vi "FixJKIHelper.vi"() -> ()   [LabVIEW 2017]
uses:
  _Support/Common/Format Timestamp.vi
  _Shared/CSM Shared.lvlib
  _csmDoc/csmdoc.lvlib
  Communicable State Machine.lvlib
  user32.dll
panel:
  out "String Cache":string
  in  "Bottom Right":string
  in  "Bottom Left":string
  out "2D Picture":picture
  in  "Error in":errorcluster caption="error in (no error)"
  out "Listbox":i32(listbox)
  in  "Progress Bar":u8(slide) scale=-1.0..226.0
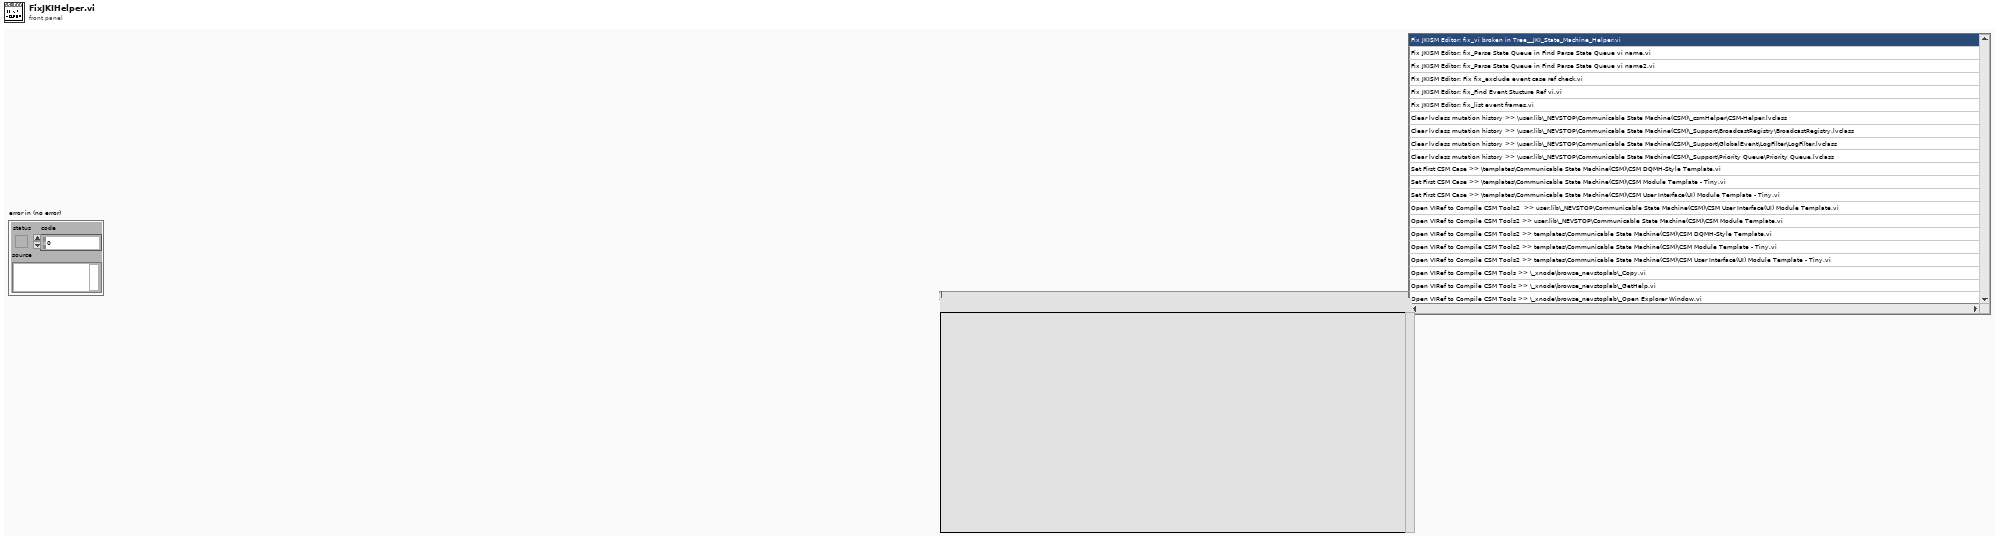
[diagram p1: front panel]
types:
  T1 = enum32{"Invalid", "Standard", "Closed", "Hidden", "Minimized", "Maximized"}
  T2 = enum32{"invalid app kind", "Development System", "Run Time System", "Student Edition", "Embedded LabVIEW", "Evaluation", "Custom"}
  T3 = cluster{"Core":cluster{"Current VI Reference":refnum<vi>, "Close Panel on Exit?":bool}, "Listbox Symbols":i32[], "Listbox Index":i32, "_JKI State Machine Helper VIs":path[], "CSM Templates":path[], "CSM lvclass":path[], "_JKI State Machine Helper Folders":path[], "Actions":string[], "LangID":string, "DescMap":variant, "NoteMap":variant, "Polish":cluster{"Version":refnum<vi>, "Action":refnum<vi>, "Progress Bar":refnum<vi>, "2D Picture":refnum<vi>, "Hold":bool, "Slides":picture[]}}
  T4 = cluster{"Version":refnum<vi>, "Action":refnum<vi>, "Progress Bar":refnum<vi>, "2D Picture":refnum<vi>, "Hold":bool, "Slides":picture[]}
  T5 = cluster{"Current VI Reference":refnum<vi>, "Close Panel on Exit?":bool}
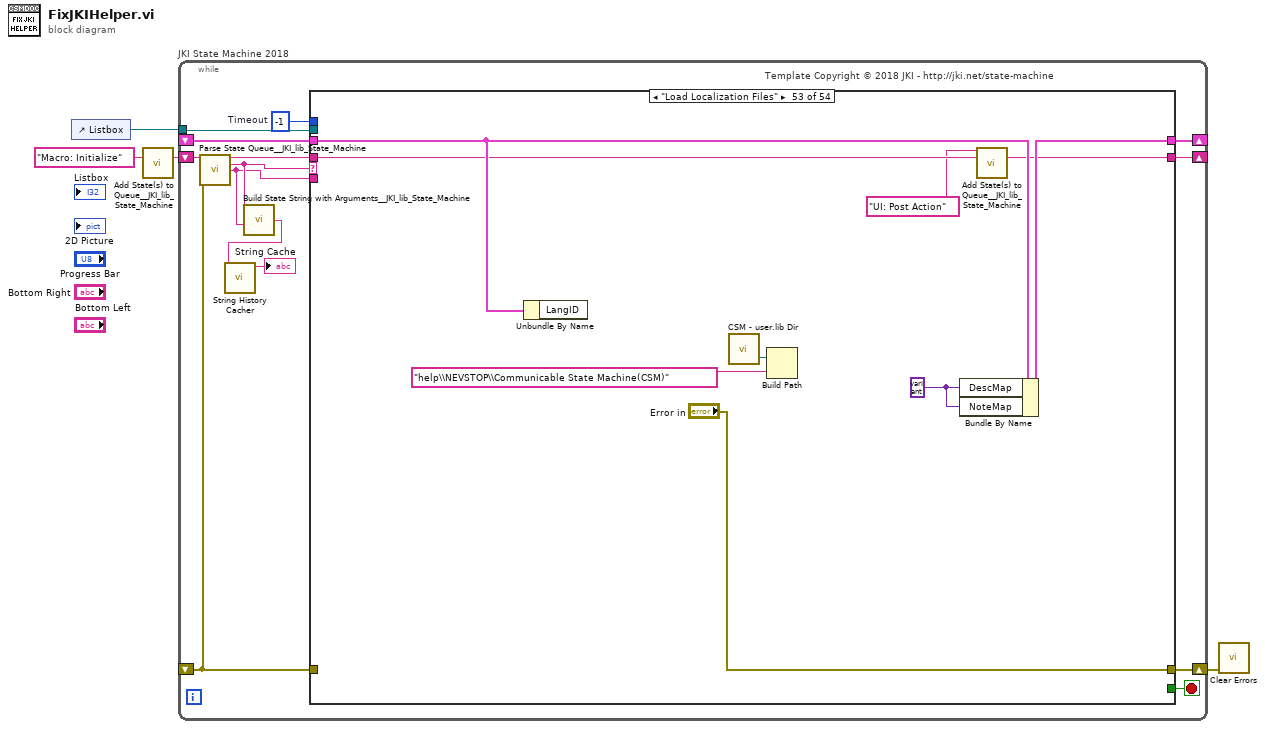
[diagram p0: block diagram]
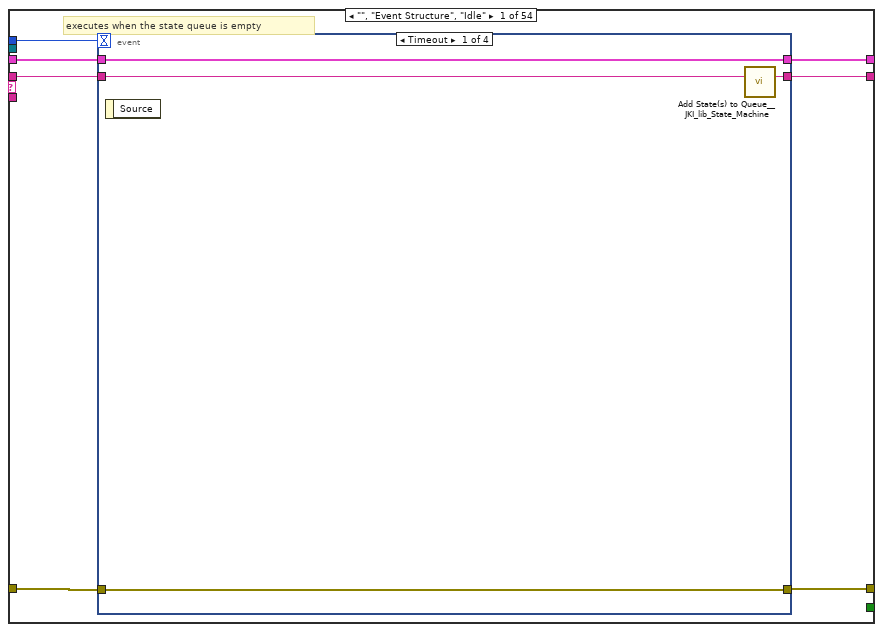
[diagram p2: hidden frame]
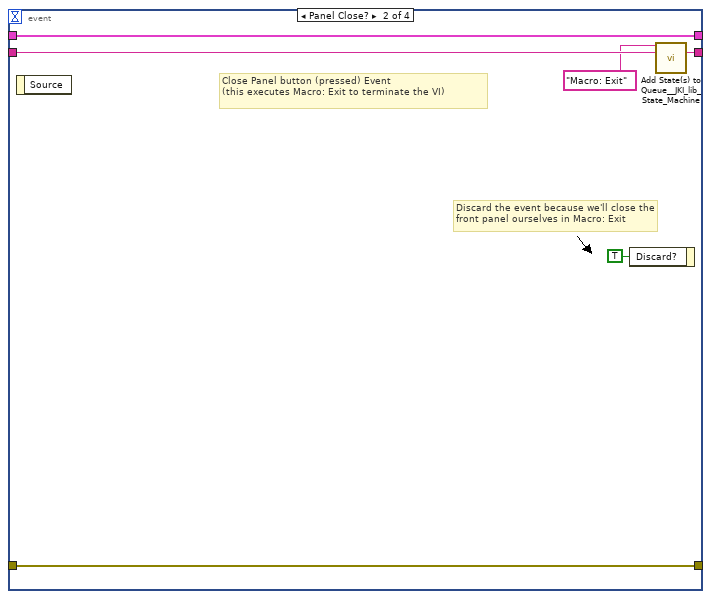
[diagram p3: hidden frame]
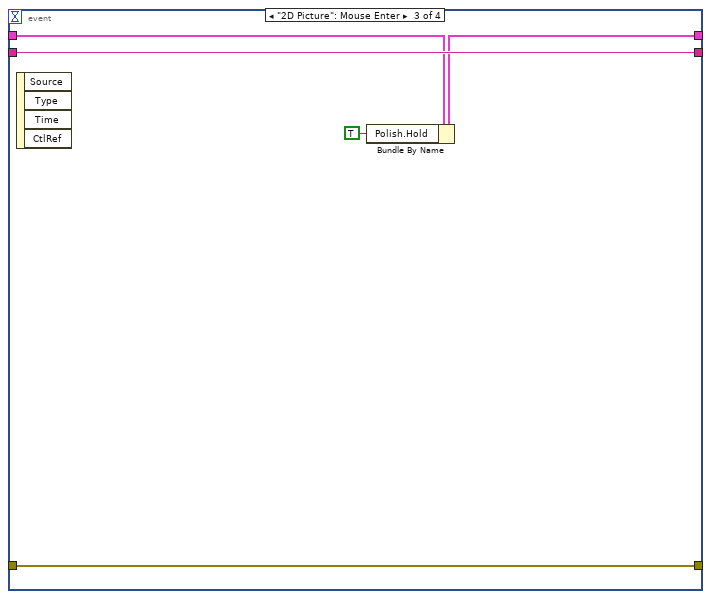
[diagram p4: hidden frame]
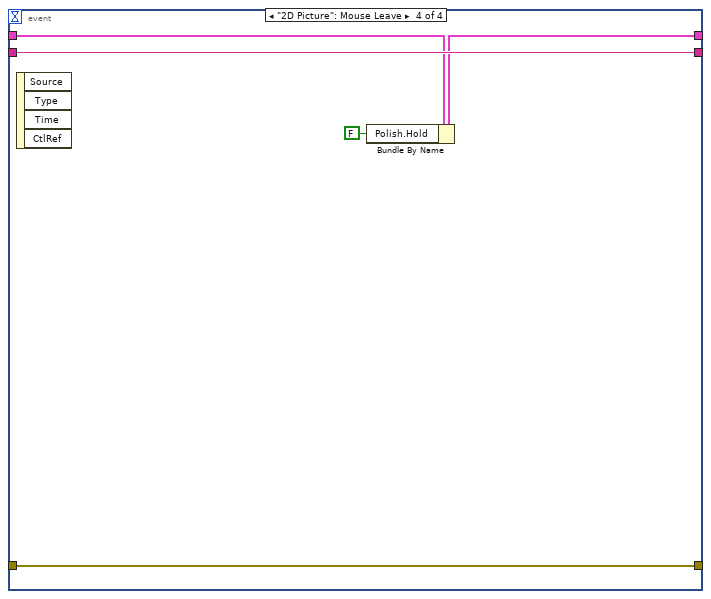
[diagram p5: hidden frame]
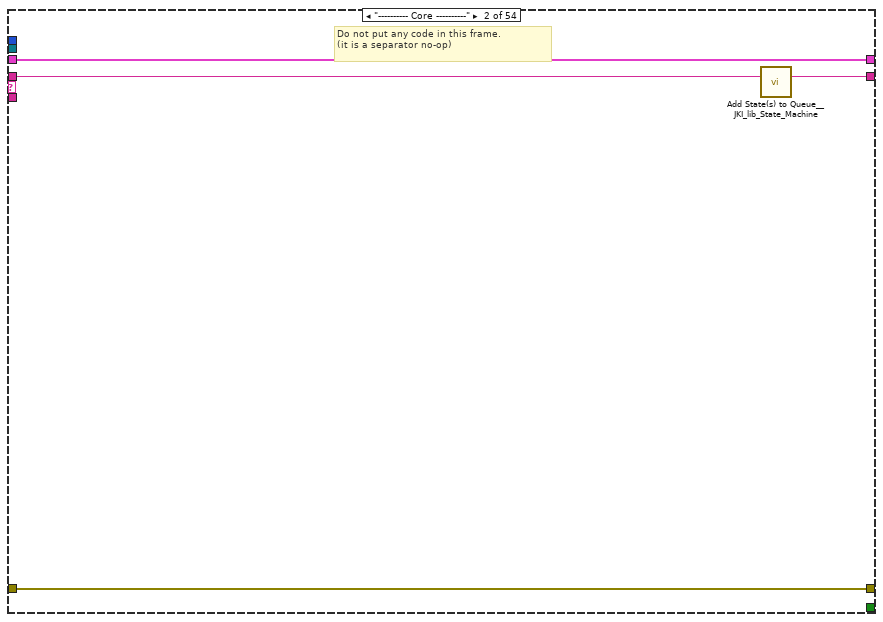
[diagram p6: hidden frame]
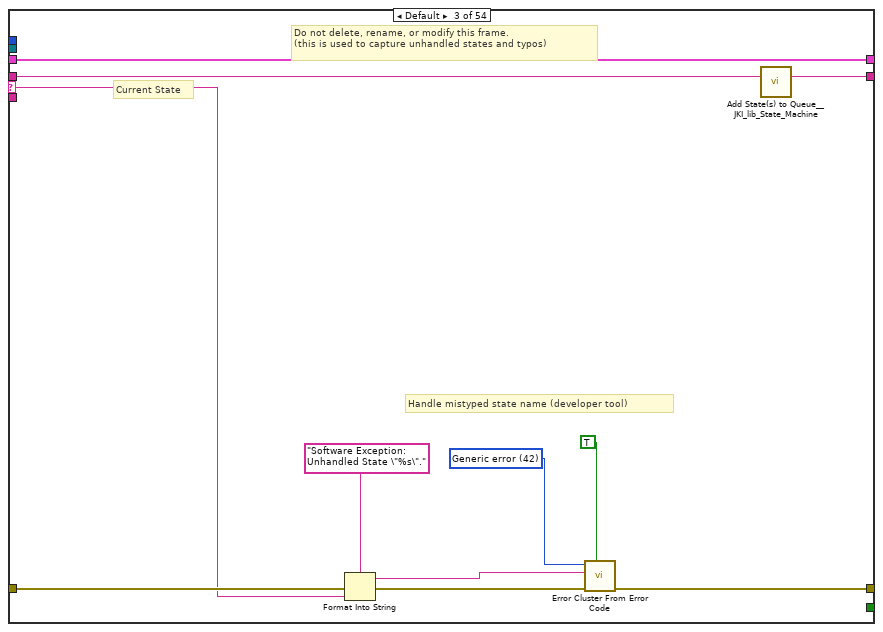
[diagram p7: hidden frame]
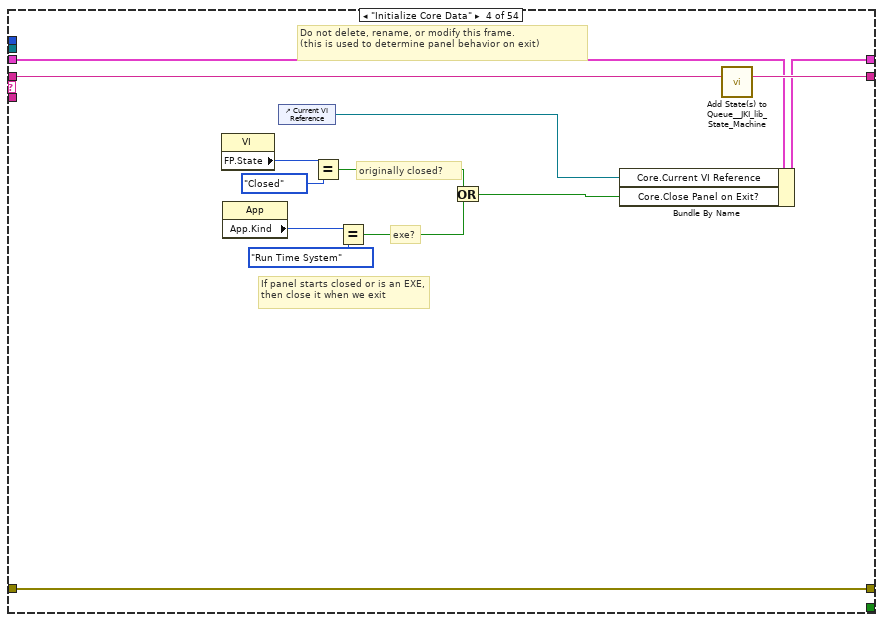
[diagram p8: hidden frame]
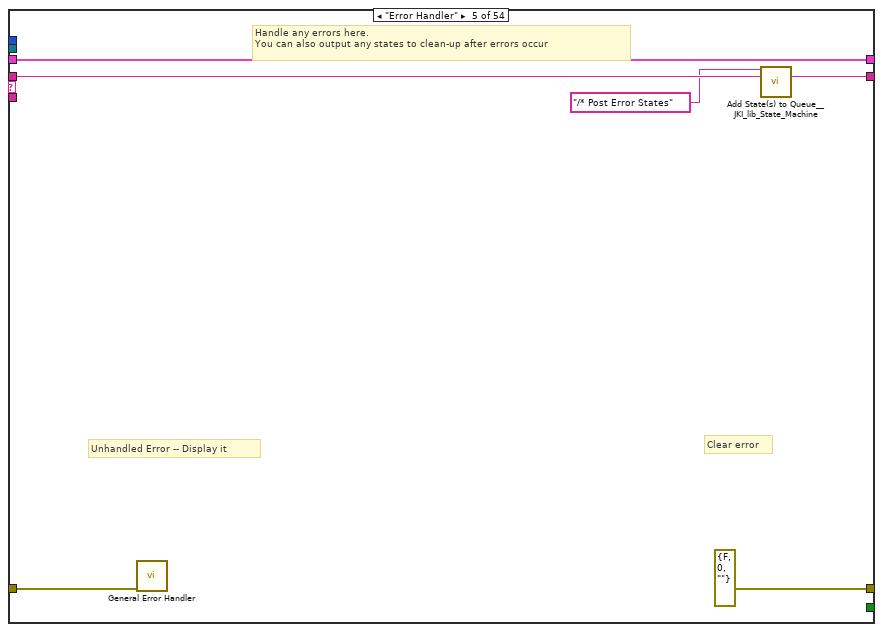
[diagram p9: hidden frame]
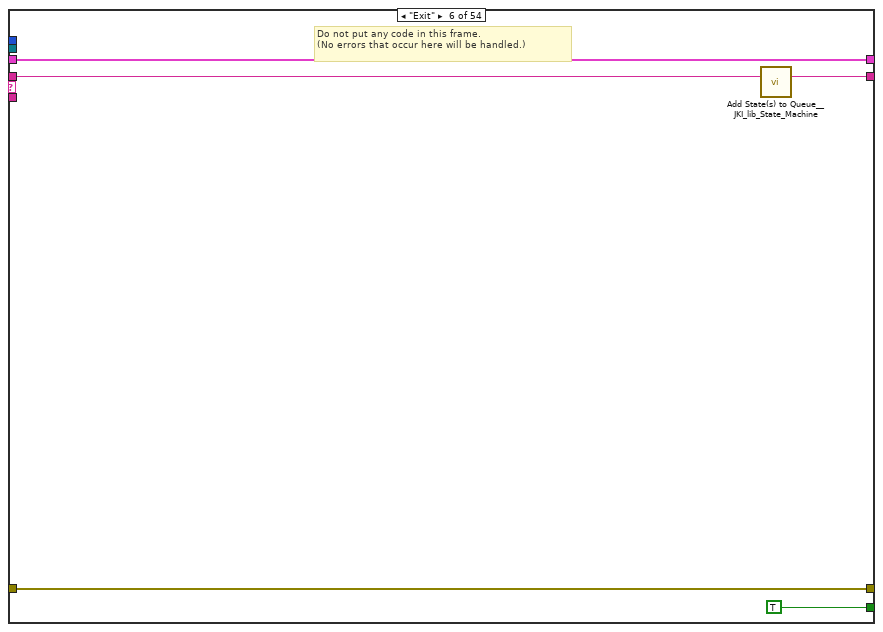
[diagram p10: hidden frame]
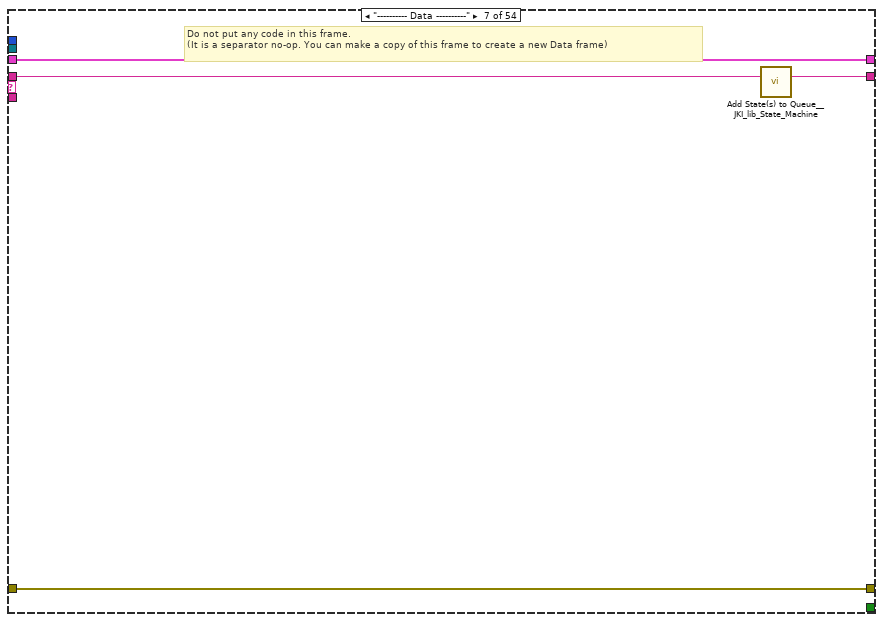
[diagram p11: hidden frame]
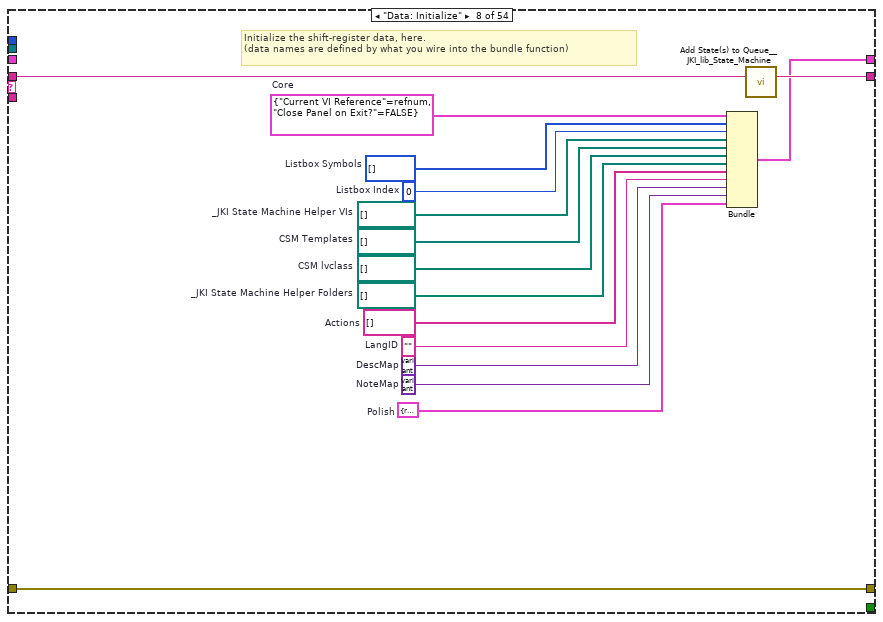
[diagram p12: hidden frame]
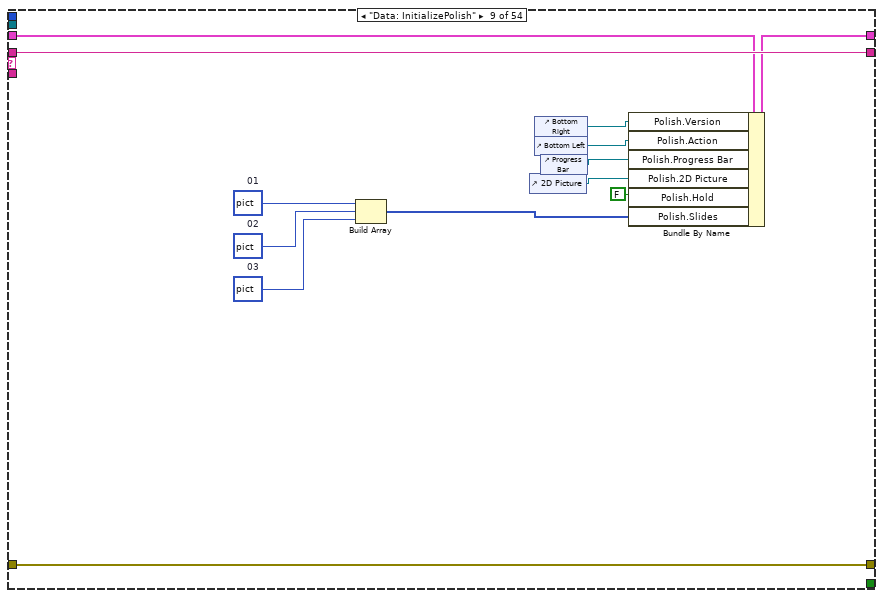
[diagram p13: hidden frame]
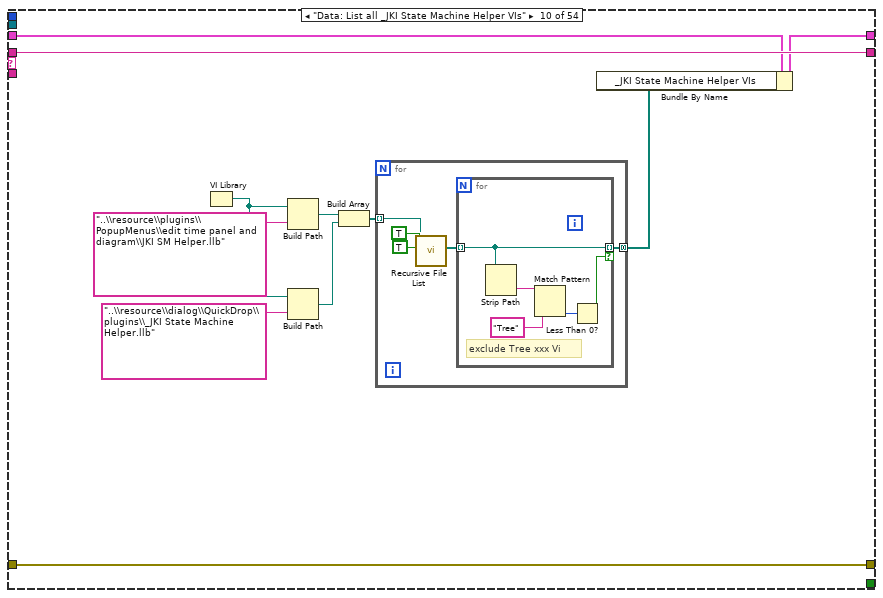
[diagram p14: hidden frame]
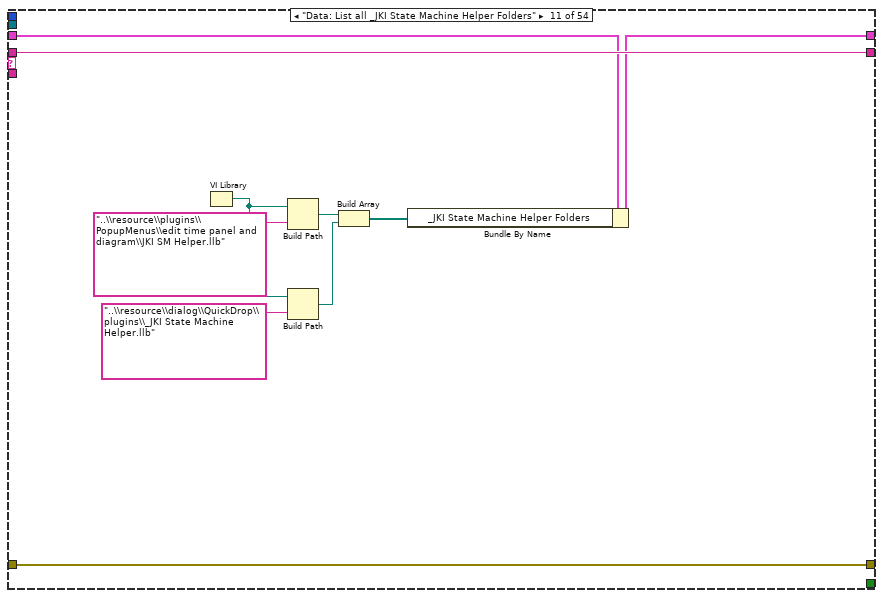
[diagram p15: hidden frame]
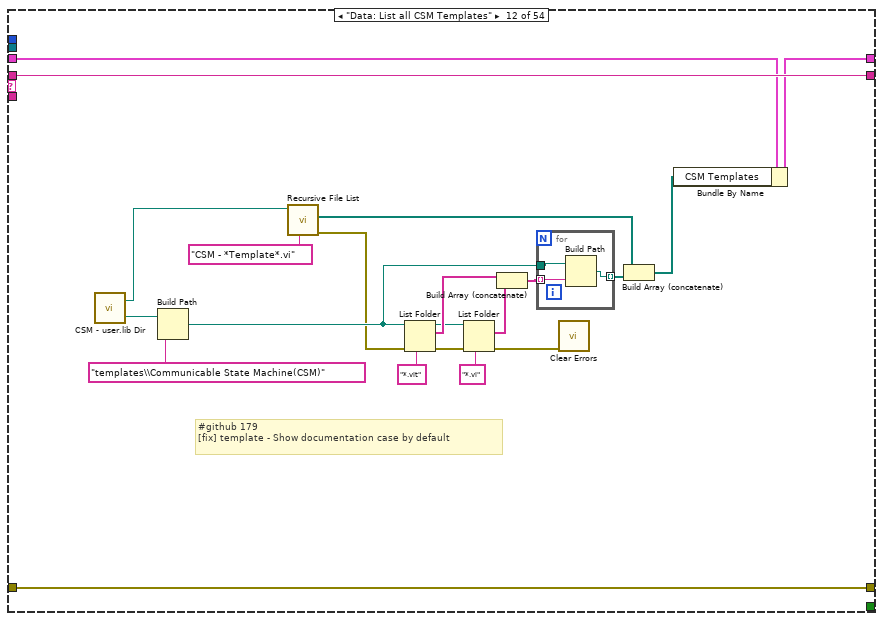
[diagram p16: hidden frame]
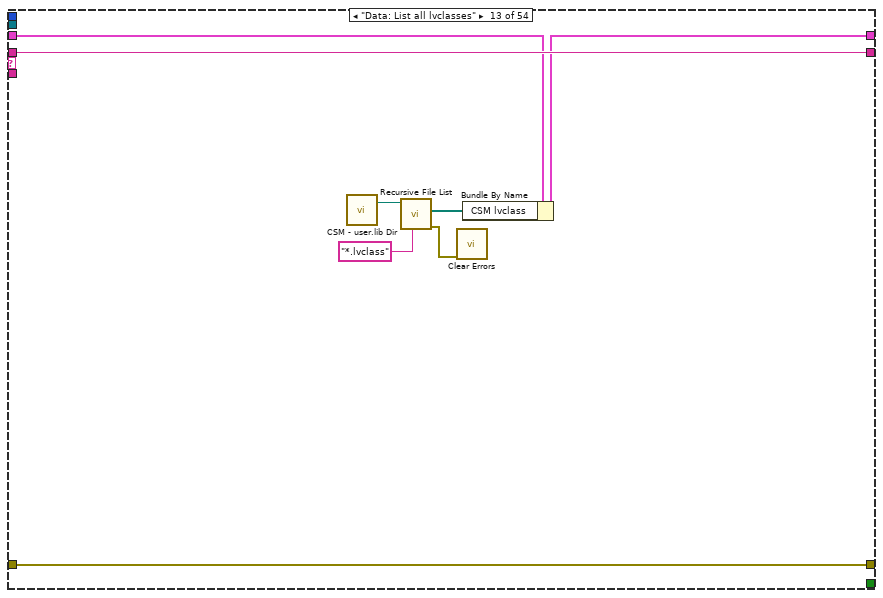
[diagram p17: hidden frame]
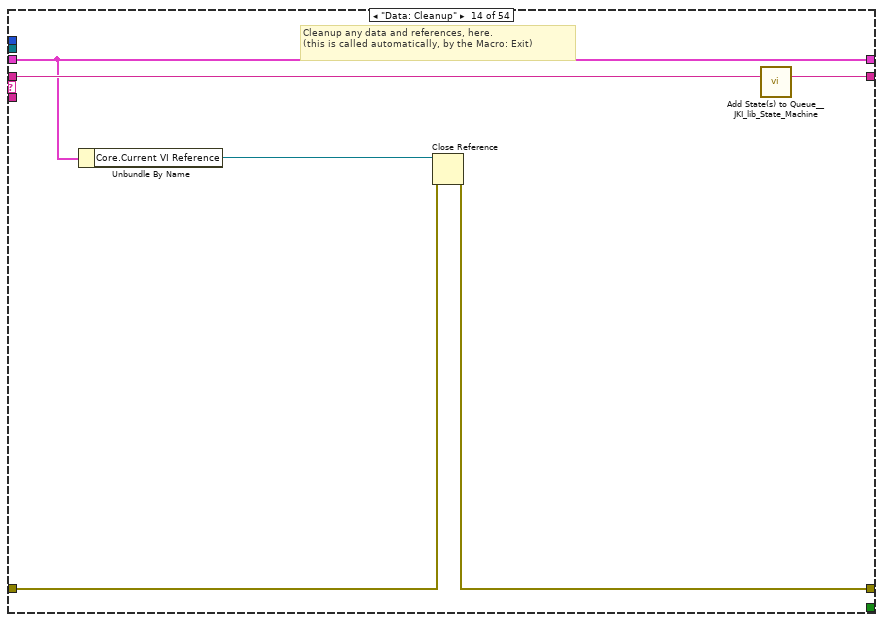
[diagram p18: hidden frame]
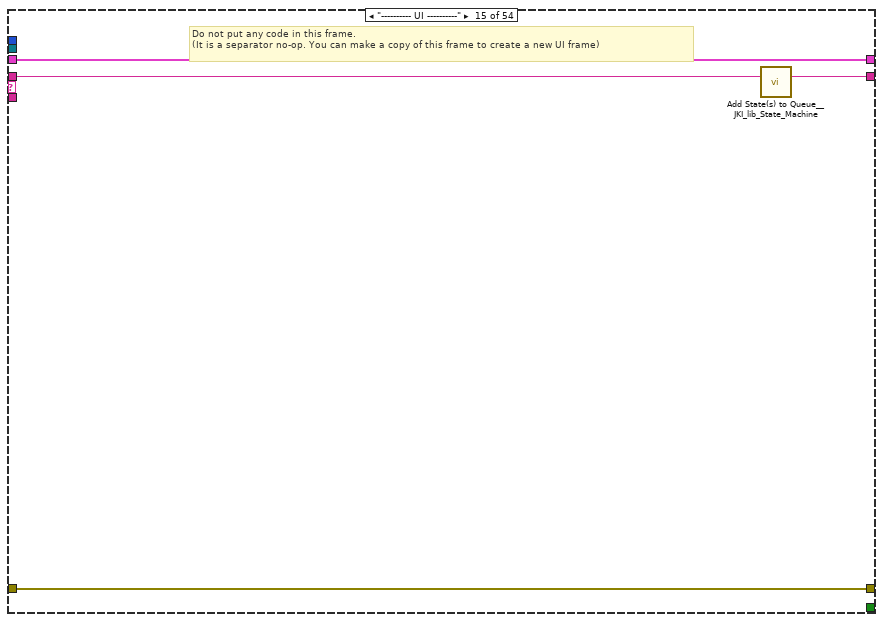
[diagram p19: hidden frame]
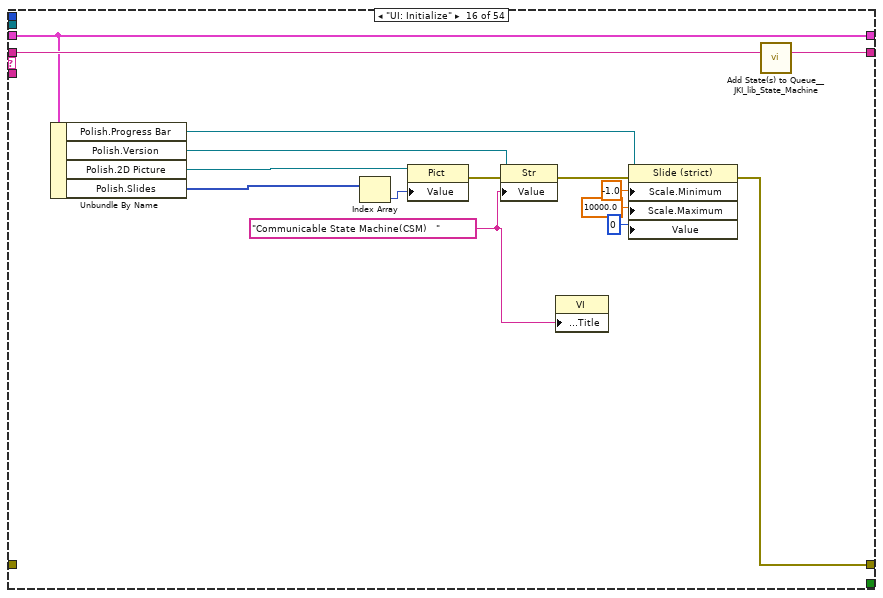
[diagram p20: hidden frame]
diagram:
  n1 = control-ref of="Listbox"() -> (w2:refnum<vi>)
  n2 = call <vilib>:"Add State(s) to Queue__JKI_lib_State_Machine.vi"("State(s) in (\"\")"="Macro: Initialize") -> ("States Out"=w4:string)  [unwired: 14 in]
  n3 = while "JKI State Machine 2018" {
    shift-right: [w13] -> _
    shift-left: _ -> [w12]
    shift-right: [w16] -> w1
    shift-left: _ -> [w10]
    shift-right: [w15] -> _
    shift-left: w4 -> [w17]
    tunnel: w2 -> [w9]
    stop <- w14 stop-if-true
    w11 = -1  # Timeout
    # "Template Copyright © 2018 JKI - http://jki.net/state-machine"
    n4 = call <vilib>:"Parse State Queue__JKI_lib_State_Machine.vi"("State Queue"=w17, "Error In (no error)"=w10) -> ("Remaining States"=w18:string, "Current State"=w7:string, "Arguments"=w6:string)  [unwired: 11 in]
    n5 = call <vilib>:"Build State String with Arguments__JKI_lib_State_Machine.vi"("Arguments (\"\")"=w6, "State"=w7) -> ("State with Arguments"=w5:string)  [unwired: 4 in]
    n6 = call "String History Cacher.vi"("String"=w5) -> ("String Cache"=→"String Cache":string)  [unwired: 10 in]
    n7 = case shown="\"Load Localization Files\"" w7 {
      selector: w7 -> [_ _ w50 _ _ _ _ _ _ _ _ _ _ _ _ _ _ _ _ _ _ _ _ _ _ _ _ _ _ _ _ _ _ _ _ _ _ _ _ _ _ _ _ _ _ _ _ _ _ _ _ _ _ _]
      tunnel: w18 -> [w25 w49 w54 w73 w79 w84 w88 w104 w116 w128 w148 w168 w179 w186 w190 w205 w215 w222 w229 w263 w330 w370 w375 w377 w391 w415 w421 w434 w436 w447 w461 w470 w487 w503 w518 w532 w545 w547 w568 w579 w584 w589 w594 w599 w604 w609 w619 w631 w661 w690 w711 w729 w737 w748]
      tunnel: w6 -> [_ _ _ _ _ _ _ _ _ _ _ _ _ _ _ _ _ w217 _ w257 _ _ _ _ _ _ _ _ _ _ _ _ _ _ w517 _ _ w550 w562 w573 _ _ _ _ _ _ w613 w626 w654 w684 _ _ _ w745]
      tunnel: w12 -> [w23 w46 w52 w66 w76 w82 w85 _ w115 w127 w147 w167 w178 w181 w187 w202 w212 w220 w227 w259 w339 w367 w372 w380 w393 w417 w423 w431 w435 w445 w459 w468 w486 w501 w515 w530 w542 w560 w571 w581 w586 w591 w596 w601 w606 w611 w622 w633 w663 w692 w719 w733 w740 w751]
      tunnel: [w22 w47 w56 w70 errorcluster {"status"=FALSE, "code"=0, "source"=""} ("error out") w81 w86 w101 w117 w118 w140 w169 w180 w182 w188 w192 w216 w218 w228 w260 w357 w368 w373 w381 w394 w418 w424 w432 w437 w443 w460 w466 w484 w499 w511 w529 w543 w561 w572 w582 w587 w592 w597 w602 w607 w612 w624 w634 w664 w693 w720 w734 "Error in" w750] -> w16
      tunnel: w10 -> [w21 w47 w55 w70 w75 w81 w86 w101 w117 w118 w140 w169 w180 w183 w188 _ w216 w219 _ w261 w357 w368 w373 w381 w394 w418 w424 w432 w437 w443 w460 w466 w484 w499 w511 w529 w543 w561 w572 w582 w587 w592 w597 w602 w607 w612 w624 w634 w664 w693 w720 w734 _ _]
      tunnel: [w24 w48 w53 w72 w78 w83 w87 w103 w116 w128 w148 w168 w179 w185 w189 w204 w215 w221 w229 w262 w331 w369 w374 w378 w392 w416 w422 w433 w436 w447 w461 w470 w487 w503 w518 w532 w544 w548 w569 w580 w585 w590 w595 w600 w605 w610 w620 w632 w662 w691 w712 w730 w738 w749] -> w15
      tunnel: [_ _ _ _ _ TRUE _ _ _ _ _ _ _ _ _ _ _ _ _ _ _ _ _ _ _ _ _ _ _ _ _ _ _ _ _ _ _ _ _ _ _ _ _ _ _ _ _ _ _ _ _ _ _ _] -> w14
      tunnel: [w20 w46 w52 w71 w76 w82 w85 w102 w114 w120 w141 w150 w175 w181 w187 w202 w212 w220 w227 w259 w339 w367 w372 w380 w393 w417 w423 w431 w435 w440 w458 w464 w481 w497 w514 w528 w542 w560 w571 w581 w586 w591 w596 w601 w606 w611 w622 w633 w663 w692 w719 w732 w739 w751] -> w13
      tunnel: w11 -> [w19 _ _ _ _ _ _ _ _ _ _ _ _ _ _ _ _ _ _ _ _ _ _ _ _ _ _ _ _ _ _ _ _ _ _ _ _ _ _ _ _ _ _ _ _ _ _ _ _ _ _ _ _ _]
      tunnel: w9 -> [_ _ _ _ _ _ _ _ _ _ _ _ _ _ _ _ w211 _ _ _ w346 _ _ _ _ _ _ _ _ _ _ _ _ _ _ _ _ _ _ _ _ _ _ _ _ _ _ _ _ _ _ _ _ _]
      frame "", "Event Structure", "Idle" {
        # "executes when the state queue is empty"
        n8 = event shown="[0] Timeout" {
          selector: _ -> [_ _ _ _]
          dyn-events: _ -> [_ _ _ _]
          timeout: w19 -> [_ _ _ _]
          tunnel: w25 -> [w29 w35 w40 w45]
          tunnel: [w28 w34 w40 w45] -> w24
          tunnel: w23 -> [w26 w32 w38 w43]
          tunnel: [w27 w33 w39 w44] -> w22
          tunnel: w21 -> [w27 w33 w39 w44]
          tunnel: [w26 w32 w36 w41] -> w20
          event Timeout {
            n9 = event-data() -> ()  [unwired: 1 in, 1 out]
            n10 = call <vilib>:"Add State(s) to Queue__JKI_lib_State_Machine.vi"("State(s) in (\"\")"=w29) -> ("States Out"=w28:string)  [unwired: 14 in]
          }
          event Panel Close? {
            # "Discard the event because we'll close the front panel ourselves in Macro: Exit"
            # "Close Panel button (pressed) Event\n(this executes Macro: Exit to terminate the VI)"
            n11 = event-data() -> ()  [unwired: 1 in, 1 out]
            n12 = event-data("Discard?"=TRUE) -> ()  [unwired: 1 in, 1 out]
            n13 = call <vilib>:"Add State(s) to Queue__JKI_lib_State_Machine.vi"("State(s) in Front (\"\")"="Macro: Exit", "State(s) in (\"\")"=w35) -> ("States Out"=w34:string)  [unwired: 13 in]
          }
          event "2D Picture": Mouse Enter {
            n14 = event-data() -> ()  [unwired: 1 in, 4 out]
            n15 = Bundle By Name(cluster=w38, "Polish.Hold"=TRUE) -> (w36:T3)
          }
          event "2D Picture": Mouse Leave {
            n16 = event-data() -> ()  [unwired: 1 in, 4 out]
            n17 = Bundle By Name(cluster=w43, "Polish.Hold"=FALSE) -> (w41:T3)
          }
        }
      }
      frame "---------- Core ----------" {
        # "Do not put any code in this frame.\n(it is a separator no-op)"
        n18 = call <vilib>:"Add State(s) to Queue__JKI_lib_State_Machine.vi"("State(s) in (\"\")"=w49) -> ("States Out"=w48:string)  [unwired: 14 in]
      }
      frame Default {
        w59 = 42 items=["No error", "Argument error", "Memory is full", "Out of zone", "End of file", "File already open", "Generic file I/O error", "File not found", "File permission error", "Disk is full", "Duplicate path", "Too many files open", "System feature not enabled", "Resource file not found", "Cannot add resource", "Resource not found", "Image not found", "Image memory error", "Pen does not exist", "Config type invalid", "Config token not found", "Config parse error", "Config memory error", "Bad external code format", "Bad external code offset", "External code not present", "Null window", "Destroy window error", "Null menu", "Print aborted", "Bad print record", "Print driver error", "Windows error during printing", "Memory error during printing", "Print dialog error", "Generic print error", "Invalid device refnum", "Device not found", "Device parameter error", "Device unit error", "Cannot open device", "Device call aborted", "Generic error", "Cancelled by user", "Object ID too low", "Object ID too high", "Object not in heap", "Unknown heap", "Unknown object (invalid DefProc)", "Unknown object (DefProc not in table)", "Message out of range", "Invalid (null) method", "Unknown message", "Manager call not supported", "Bad address", "Network operation in progress", "Network operation timed out", "Connection is busy", "Network attribute not supported", "Network error", "Address in use", "System out of memory", "Connection aborted", "Connection refused", "Not connected", "Already connected", "Connection closed", "Initialization error (interapplication manager)", "Bad occurrence", "Wait on unbound occurrence handler", "Occurrence queue overflow", "Datalog type conflict", "Unused", "Unrecognized type (interapplication manager)", "Memory corrupt", "Failed to make temporary DLL", "Old CIN version", "Drag socket not found", "Failed to load drop-object", "Failed to register OLE object", "Failed to release OLE object", "Format specifier type mismatch", "Unknown format specifier", "Too few format specifiers", "Too many format specifiers", "Scan failed", "Newer CIN version", "Error converting to variant", "Runtime menu error", "Password tampered", "Variant attribute not found", "Incompatible variant data type", "Event data is not available", "Event Store is not present", "Occurrence is not found", "Event Queue is not created", "Event info is not available", "Refnum passed is NULL", "Error retrieving Class GUID", "Error retrieving CoClass GUID", "Error retrieving TypeLib GUID.", "Bad built application magic bytes.", "Specific driver is different from the specific driver associated with the Logical Name.", "There is no session opened to the class driver.", "Max Error", "MAX - Error with config objects", "MAX - Error loading configuration", "MAX - Group not supported"]
        # "Current State"
        # "Do not delete, rename, or modify this frame.\n(this is used to capture unhandled states and typos)"
        # "Handle mistyped state name (developer tool)"
        n19 = Format Into String(format string="Software Exception: Unhandled State \"%s\"." ("message"), error in=w55, w50) -> (resulting string=w58:string, error out=w57:errorcluster)  [unwired: 1 in]
        n20 = call <vilib>:"Error Cluster From Error Code.vi"("show call chain? (False)"=TRUE, "error in (no error)"=w57, "error message (\"\")"=w58, "error code (0)"=w59) -> ("error out"=w56:errorcluster)  [unwired: 5 in]
        n21 = call <vilib>:"Add State(s) to Queue__JKI_lib_State_Machine.vi"("State(s) in (\"\")"=w54) -> ("States Out"=w53:string)  [unwired: 14 in]
      }
      frame "Initialize Core Data" {
        # "Do not delete, rename, or modify this frame.\n(this is used to determine panel behavior on exit)"
        # "originally closed?"
        # "exe?"
        # "If panel starts closed or is an EXE, then close it when we exit"
        n22 = property class="VI"() -> ("FP.State"=w63:T1)  [unwired: 2 in, 2 out]
        n23 = property class="App"() -> ("App.Kind"=w69:T2)  [unwired: 2 in, 2 out]
        n24 = control-ref of="Current VI Reference"() -> (w64:refnum<vi>)
        n25 = Equal?(x=w63, y=T1."Closed" ("Front Panel Window:State")) -> (x = y?=w61:bool)
        n26 = Equal?(x=w69, y=T2."Run Time System" ("Application:Kind")) -> (x = y?=w67:bool)
        n27 = Or(x=w61, y=w67) -> (x .or. y?=w65:bool)
        n28 = Bundle By Name(cluster=w66, "Core.Current VI Reference"=w64, "Core.Close Panel on Exit?"=w65) -> (w71:T3)
        n29 = call <vilib>:"Add State(s) to Queue__JKI_lib_State_Machine.vi"("State(s) in (\"\")"=w73) -> ("States Out"=w72:string)  [unwired: 14 in]
      }
      frame "Error Handler" {
        # "Unhandled Error -- Display it"
        # "Handle any errors here.\nYou can also output any states to clean-up after errors occur"
        # "Clear error"
        n30 = call <vilib>:"General Error Handler.vi"("error in (no error)"=w75) -> ()  [unwired: 10 in, 5 out]
        n31 = call <vilib>:"Add State(s) to Queue__JKI_lib_State_Machine.vi"("State(s) in Front (\"\")"="/* Post Error States", "State(s) in (\"\")"=w79) -> ("States Out"=w78:string)  [unwired: 13 in]
      }
      frame "Exit" {
        # "Do not put any code in this frame.\n(No errors that occur here will be handled.)"
        n32 = call <vilib>:"Add State(s) to Queue__JKI_lib_State_Machine.vi"("State(s) in (\"\")"=w84) -> ("States Out"=w83:string)  [unwired: 14 in]
      }
      frame "---------- Data ----------" {
        # "Do not put any code in this frame.\n(It is a separator no-op. You can make a copy of this frame to create a new Data frame)"
        n33 = call <vilib>:"Add State(s) to Queue__JKI_lib_State_Machine.vi"("State(s) in (\"\")"=w88) -> ("States Out"=w87:string)  [unwired: 14 in]
      }
      frame "Data: Initialize" {
        w89 = T4 {"Version"=refnum, "Action"=refnum, "Progress Bar"=refnum, "2D Picture"=refnum, "Hold"=TRUE, "Slides"=[]}  # Polish
        w90 = variant  # NoteMap
        w91 = variant  # DescMap
        w92 = ""  # LangID
        w93 = string[] []  # Actions
        w94 = path[] []  # _JKI State Machine Helper Folders
        w95 = path[] []  # CSM lvclass
        w96 = i32[] []  # Listbox Symbols
        w97 = 0  # Listbox Index
        w98 = path[] []  # CSM Templates
        w99 = path[] []  # _JKI State Machine Helper VIs
        w100 = T5 {"Current VI Reference"=refnum, "Close Panel on Exit?"=FALSE}  # Core
        # "Initialize the shift-register data, here.\n(data names are defined by what you wire into the bundle function)"
        n34 = Bundle("Core"=w100, "Listbox Symbols"=w96, "Listbox Index"=w97, "_JKI State Machine Helper VIs"=w99, "CSM Templates"=w98, "CSM lvclass"=w95, "_JKI State Machine Helper Folders"=w94, "Actions"=w93, "LangID"=w92, "DescMap"=w91, "NoteMap"=w90, "Polish"=w89) -> (w102:T3)  [unwired: 1 in]
        n35 = call <vilib>:"Add State(s) to Queue__JKI_lib_State_Machine.vi"("State(s) in (\"\")"=w104) -> ("States Out"=w103:string)  [unwired: 14 in]
      }
      frame "Data: InitializePolish" {
        w105 = picture bytes[1036830]  # 03
        w106 = picture bytes[1036830]  # 02
        w107 = picture bytes[1036830]  # 01
        n36 = Build Array(w107, w106, w105) -> (w110:picture[])
        n37 = control-ref of="2D Picture"() -> (w112:refnum<vi>)
        n38 = control-ref of="Bottom Right"() -> (w109:refnum<vi>)
        n39 = control-ref of="Bottom Left"() -> (w108:refnum<vi>)
        n40 = control-ref of="Progress Bar"() -> (w113:refnum<vi>)
        n41 = Bundle By Name(cluster=w115, "Polish.Version"=w109, "Polish.Action"=w108, "Polish.Progress Bar"=w113, "Polish.2D Picture"=w112, "Polish.Hold"=FALSE, "Polish.Slides"=w110) -> (w114:T3)
      }
      frame "Data: List all _JKI State Machine Helper VIs" {
        n42 = VI Library() -> (path=w125:path)
        n43 = Build Path(base path=w125, name or relative path="..\\resource\\plugins\\PopupMenus\\edit time panel and diagram\\JKI SM Helper.llb") -> (appended path=w123:path)
        n44 = Build Path(base path=w125, name or relative path="..\\resource\\dialog\\QuickDrop\\plugins\\_JKI State Machine Helper.llb") -> (appended path=w121:path)
        n45 = Build Array(w123, w121) -> (w122:path[])
        n46 = for {
          tunnel: w122 -> [w131] mode=indexing
          tunnel: [w129] -> w119 mode=concatenating
          n47 = call <vilib>:"Recursive File List.vi"("Continue Recursing on Error? (F)"=TRUE, "Treat LLBs as Folders?"=TRUE, "Folder Path"=w131) -> ("All Files in Dir"=w130:path[])  [unwired: 4 in, 4 out]
          n48 = for {
            tunnel: w130 -> [w135] mode=indexing
            tunnel: [w135] -> w129 mode=indexing if=w134
            # "exclude Tree xxx Vi"
            n49 = Strip Path(path=w135) -> (name=w138:string)  [unwired: 1 out]
            n50 = Match Pattern(string=w138, regular expression="Tree") -> (offset past match=w136:i32)  [unwired: 1 in, 3 out]
            n51 = Less Than 0?(x=w136) -> (x < 0?=w134:bool)
          }
        }
        n52 = Bundle By Name(cluster=w127, "_JKI State Machine Helper VIs"=w119) -> (w120:T3)
      }
      frame "Data: List all _JKI State Machine Helper Folders" {
        n53 = VI Library() -> (path=w145:path)
        n54 = Build Path(base path=w145, name or relative path="..\\resource\\plugins\\PopupMenus\\edit time panel and diagram\\JKI SM Helper.llb") -> (appended path=w143:path)
        n55 = Build Path(base path=w145, name or relative path="..\\resource\\dialog\\QuickDrop\\plugins\\_JKI State Machine Helper.llb") -> (appended path=w142:path)
        n56 = Build Array(w143, w142) -> (w139:path[])
        n57 = Bundle By Name(cluster=w147, "_JKI State Machine Helper Folders"=w139) -> (w141:T3)
      }
      frame "Data: List all CSM Templates" {
        # "#github 179\n[fix] template - Show documentation case by default"
        n58 = call "CSM - user.lib Dir.vi"() -> ("<LabVIEW>"=w157:path, "csm_user.lib_dir"=w159:path)  [unwired: 2 in]
        n59 = Build Path(base path=w157, name or relative path="templates\\Communicable State Machine(CSM)") -> (appended path=w166:path)
        n60 = call <vilib>:"Recursive File List.vi"("pattern"="CSM - *Template*.vi" ("name or relative path"), "Folder Path"=w159) -> ("error out"=w160:errorcluster, "All Files in Dir"=w161:path[])  [unwired: 5 in, 3 out]
        n61 = List Folder(path=w166, pattern="*.vit", error in=w160) -> (path out=w153:path, filenames=w162:string[], error out=w155:errorcluster)  [unwired: 1 in, 1 out]
        n62 = List Folder(path=w153, pattern="*.vi", error in=w155) -> (filenames=w163:string[], error out=w156:errorcluster)  [unwired: 1 in, 2 out]
        n63 = Build Array (concatenate)(w162, w163) -> (w164:string[])
        n64 = for {
          tunnel: w164 -> [w172] mode=indexing
          tunnel: [w171] -> w165 mode=indexing
          tunnel: w166 -> [w170]
          n65 = Build Path(base path=w170, name or relative path=w172) -> (appended path=w171:path)
        }
        n66 = call <vilib>:"Clear Errors.vi"("error in (no error)"=w156) -> ()  [unwired: 5 in, 2 out]
        n67 = Build Array (concatenate)(w161, w165) -> (w149:path[])
        n68 = Bundle By Name(cluster=w167, "CSM Templates"=w149) -> (w150:T3)
      }
      frame "Data: List all lvclasses" {
        n69 = call "CSM - user.lib Dir.vi"() -> ("csm_user.lib_dir"=w177:path)  [unwired: 2 in, 1 out]
        n70 = call <vilib>:"Recursive File List.vi"("pattern"="*.lvclass", "Folder Path"=w177) -> ("error out"=w173:errorcluster, "All Files in Dir"=w174:path[])  [unwired: 5 in, 3 out]
        n71 = call <vilib>:"Clear Errors.vi"("error in (no error)"=w173) -> ()  [unwired: 5 in, 2 out]
        n72 = Bundle By Name(cluster=w178, "CSM lvclass"=w174) -> (w175:T3)
      }
      frame "Data: Cleanup" {
        # "Cleanup any data and references, here.\n(this is called automatically, by the Macro: Exit)"
        n73 = Unbundle By Name(w181) -> ("Core.Current VI Reference"=w184:refnum<vi>)
        n74 = Close Reference(reference=w184, error in (no error)=w183) -> (error out=w182:errorcluster)
        n75 = call <vilib>:"Add State(s) to Queue__JKI_lib_State_Machine.vi"("State(s) in (\"\")"=w186) -> ("States Out"=w185:string)  [unwired: 14 in]
      }
      frame "---------- UI ----------" {
        # "Do not put any code in this frame.\n(It is a separator no-op. You can make a copy of this frame to create a new UI frame)"
        n76 = call <vilib>:"Add State(s) to Queue__JKI_lib_State_Machine.vi"("State(s) in (\"\")"=w190) -> ("States Out"=w189:string)  [unwired: 14 in]
      }
      frame "UI: Initialize" {
        w191 = "Communicable State Machine(CSM)   " ("Value")
        n77 = Unbundle By Name(w202) -> ("Polish.Progress Bar"=w196:refnum<vi>, "Polish.Version"=w199:refnum<vi>, "Polish.2D Picture"=w201:refnum<vi>, "Polish.Slides"=w203:picture[])
        n78 = Index Array(array=w203) -> (element=w200:picture)  [unwired: 1 in]
        n79 = property class="Pict"(reference=w201, "Value"=w200) -> (error out=w198:errorcluster)  [unwired: 1 in, 1 out]
        n80 = property class="Str"(reference=w199, error in=w198, "Value"=w191) -> (error out=w197:errorcluster)  [unwired: 1 out]
        n81 = property class="VI"("Front Panel.Title"=w191) -> ()  [unwired: 2 in, 2 out]
        n82 = property class="Slide (strict)"(reference=w196, error in=w197, "Scale.Minimum"=-1.0 ("Scale.Range:Minimum"), "Scale.Maximum"=10000.0 ("Scale.Range:Maximum"), "Value"=u8 0) -> (error out=w192:errorcluster)  [unwired: 1 out]
        n83 = call <vilib>:"Add State(s) to Queue__JKI_lib_State_Machine.vi"("State(s) in (\"\")"=w205) -> ("States Out"=w204:string)  [unwired: 14 in]
      }
      frame "UI: Refresh Listbox" {
        w210 = 0 ("Top Row")
        n84 = Unbundle By Name(w212) -> ("Actions"=w208:string[], "Polish.Progress Bar"=w206:refnum<vi>)
        n85 = Array Size(array=w208) -> (size(s)=w207:i32)
        n86 = Initialize Array(0 ("Top Row"), w207) -> (w213:i32[])
        n87 = To Double Precision Float(number=w207) -> (double precision float=w209:dbl)
        n88 = property on="Property Node" class="LstBox (strict)"(reference=w211, "Item Names"=w208, "Top Row"=w210, "Item Symbols"=w213, "Value"=w210) -> ()  [unwired: 1 in, 2 out]
        n89 = property class="Slide (strict)"(reference=w206, "Scale.Maximum"=w209) -> ()  [unwired: 1 in, 2 out]
      }
      frame "UI: Cursor Set" {
        # "Argument"
        # "Set and Unset Cursor Busy.\n(Usage: \"UI: Cursor Set >> Busy|Idle\")"
        n90 = case shown="\"Idle\", Default" w217 {
          tunnel: w219 -> [w224 w226]
          tunnel: [w223 w225] -> w218
          frame "Idle", Default {
            n91 = call <vilib>:"Unset Busy.vi"("error in (no error)"=w224) -> ("error out"=w223:errorcluster)  [unwired: 10 in]
          }
          frame "Busy" {
            n92 = call <vilib>:"Set Busy.vi"("error in (no error)"=w226) -> ("error out"=w225:errorcluster)  [unwired: 9 in, 1 out]
          }
        }
        n93 = call <vilib>:"Add State(s) to Queue__JKI_lib_State_Machine.vi"("State(s) in (\"\")"=w222) -> ("States Out"=w221:string)  [unwired: 14 in]
      }
      frame "UI: Bring Window to Topmost(Windows Only)" {
        n94 = disable-structure shown="OS==Win" {
          disable-tunnel: [w235 _] -> w228
          disable-tunnel: w227 -> [w234 _]
          frame condition #0 (active) {
            w240 = 0 items=["NULL"]
            # "How to Bring the Front Panel in Front of All Desktop Windows? -Batch File Method\nhttps://knowledge.ni.com/KnowledgeArticleDetails?id=kA03q000000YOu6CAG&l=en-US"
            n95 = Unbundle By Name(w234) -> ("Core.Current VI Reference"=w233:refnum<vi>)
            n96 = property class="VI"(reference=w233) -> (error out=w236:errorcluster, "Front Panel.Title"=w237:string)  [unwired: 1 in, 1 out]
            n97 = call "CSM - user.lib Dir.vi"() -> ("csm_user.lib_dir"=w232:path)  [unwired: 2 in, 1 out]
            n98 = dll-call lib="user32.dll" fn="FindWindowA" label="FindWindow"(error in=w236, "lpszClassName"=w240, "lpszWindowName"=w237) -> (error out=w239:errorcluster, "hWnd"=w238:u64)  [unwired: 3 in, 2 out]
            n99 = Build Path(base path=w232, name or relative path="_scripts\\sendkeys.bat") -> (appended path=w230:path)
            n100 = case shown="Default" w238 {
              selector: w238 -> [_ w247]
              tunnel: w239 -> [w241 w248]
              tunnel: [w241 w246] -> w235
              tunnel: w230 -> [_ w244]
              frame 0 {
              }
              frame Default {
                n101 = dll-call lib="user32.dll" fn="SetForegroundWindow"(error in=w248, "Handle"=w247) -> (error out=w245:errorcluster)  [unwired: 3 in, 2 out]
                n102 = call <vilib>:"Check if File or Folder Exists.vi"("path"=w244) -> ("file or folder exists?"=w242:bool, "dup path"=w243:path)  [unwired: 8 in, 1 out]
                n103 = case shown="True" w242 {
                  tunnel: [w249 w254] -> w246
                  tunnel: w245 -> [w249 w253]
                  tunnel: w243 -> [_ w250]
                  frame False {
                  }
                  frame True {
                    n104 = Format Into String(format string="\"%s\" \"LabVIEW\" \"\"" ("command line"), w250) -> (resulting string=w251:string)  [unwired: 2 in, 1 out]
                    n105 = call <vilib>:"System Exec.vi"("run minimized? (F)"=TRUE, "wait until completion? (T)"=TRUE, "error in (no error)"=w253, "command line"=w251) -> ("error out"=w254:errorcluster)  [unwired: 4 in, 3 out]
                  }
                }
              }
            }
          }
          frame condition #1 {
          }
        }
      }
      frame "UI: Front Panel State" {
        # "Argument"
        # "Set Front Panel Open or Closed\n(Usage: \"UI: Front Panel State >> Open|Close\")"
        n106 = Unbundle By Name(w259) -> ("Core.Current VI Reference"=w258:refnum<vi>)
        n107 = case shown="\"Minimize\", \"Minimized\"" w257 {
          tunnel: w261 -> [w269 w284 w295 w308 w321]
          tunnel: [w271 w285 w297 w310 w323] -> w260
          tunnel: w258 -> [w270 w282 w296 w309 w322]
          frame "Open", "Standard", Default {
            w264 = T1."Standard" ("State")
            n108 = property class="VI"(reference=w270, error in=w269) -> (reference out=w267:refnum<vi>, error out=w268:errorcluster, "FP.State"=w266:T1)
            n109 = Not Equal?(x=w266, y=w264) -> (x != y?=w265:bool)
            n110 = case shown="True" w265 {
              tunnel: [w275 w277] -> w271
              tunnel: w268 -> [w274 w277]
              tunnel: w267 -> [w273 _]
              tunnel: w264 -> [w272 _]
              frame True {
                n111 = invoke class="VI" method="FP.Open"(reference=w273, error in=w274, "Activate"=TRUE, "State"=w272) -> (error out=w275:errorcluster)  [unwired: 1 in, 4 out]
              }
              frame False {
              }
            }
          }
          frame "Close", "Closed" {
            n112 = property class="VI"(reference=w282, error in=w284) -> (reference out=w281:refnum<vi>, error out=w283:errorcluster, "FP.State"=w279:T1)
            n113 = Not Equal?(x=w279, y=T1."Closed" ("Front Panel Window:State")) -> (x != y?=w278:bool)
            n114 = case shown="True" w278 {
              tunnel: [w286 w289] -> w285
              tunnel: w283 -> [w286 w288]
              tunnel: w281 -> [_ w287]
              frame False {
              }
              frame True {
                n115 = invoke class="VI" method="FP.Close"(reference=w287, error in=w288) -> (error out=w289:errorcluster)  [unwired: 1 in, 2 out]
              }
            }
          }
          frame "Hidden", "Hide" {
            w290 = T1."Hidden" ("State")
            n116 = property class="VI"(reference=w296, error in=w295) -> (reference out=w293:refnum<vi>, error out=w294:errorcluster, "FP.State"=w292:T1)
            n117 = Not Equal?(x=w292, y=w290) -> (x != y?=w291:bool)
            n118 = case shown="True" w291 {
              tunnel: [w301 w302] -> w297
              tunnel: w294 -> [w300 w302]
              tunnel: w293 -> [w299 _]
              tunnel: w290 -> [w298 _]
              frame True {
                n119 = invoke class="VI" method="FP.Open"(reference=w299, error in=w300, "State"=w298) -> (error out=w301:errorcluster)  [unwired: 2 in, 4 out]
              }
              frame False {
              }
            }
          }
          frame "Minimize", "Minimized" {
            w303 = T1."Minimized" ("State")
            n120 = property class="VI"(reference=w309, error in=w308) -> (reference out=w306:refnum<vi>, error out=w307:errorcluster, "FP.State"=w305:T1)
            n121 = Not Equal?(x=w305, y=w303) -> (x != y?=w304:bool)
            n122 = case shown="True" w304 {
              tunnel: [w314 w315] -> w310
              tunnel: w307 -> [w313 w315]
              tunnel: w306 -> [w312 _]
              tunnel: w303 -> [w311 _]
              frame True {
                n123 = invoke class="VI" method="FP.Open"(reference=w312, error in=w313, "State"=w311) -> (error out=w314:errorcluster)  [unwired: 2 in, 4 out]
              }
              frame False {
              }
            }
          }
          frame "Maximize", "Maximized" {
            w316 = T1."Maximized" ("State")
            n124 = property class="VI"(reference=w322, error in=w321) -> (reference out=w319:refnum<vi>, error out=w320:errorcluster, "FP.State"=w318:T1)
            n125 = Not Equal?(x=w318, y=w316) -> (x != y?=w317:bool)
            n126 = case shown="True" w317 {
              tunnel: [w327 w328] -> w323
              tunnel: w320 -> [w326 w328]
              tunnel: w319 -> [w325 _]
              tunnel: w316 -> [w324 _]
              frame True {
                n127 = invoke class="VI" method="FP.Open"(reference=w325, error in=w326, "State"=w324) -> (error out=w327:errorcluster)  [unwired: 2 in, 4 out]
              }
              frame False {
              }
            }
          }
        }
        n128 = call <vilib>:"Add State(s) to Queue__JKI_lib_State_Machine.vi"("State(s) in (\"\")"=w263) -> ("States Out"=w262:string)  [unwired: 14 in]
      }
      frame "UI: Post Action" {
        n129 = Unbundle By Name(w339) -> ("Polish.Hold"=w337:bool, "Polish.2D Picture"=w335:refnum<vi>, "Polish.Slides"=w334:picture[], "Polish.Action"=w342:refnum<vi>, "Polish.Progress Bar"=w344:refnum<vi>)
        n130 = property on="Property Node" class="LstBox (strict)"(reference=w346) -> (reference out=w348:refnum<vi>, error out=w347:errorcluster, "Value"=w338:i32, "Item Symbols"=w356:i32[], "Item Names"=w345:string[])  [unwired: 1 in]
        n131 = call "Periodic Trigger (OpenG).vi"("Time (ms)"=u32 3000 ("time (ms)")) -> ("Triggered"=w332:bool)  [unwired: 12 in, 2 out]
        n132 = Not(x=w337) -> (.not. x?=w340:bool)
        n133 = And(x=w332, y=w340) -> (x .and. y?=w336:bool)
        n134 = case shown="True" w336 {
          tunnel: w335 -> [_ w366]
          tunnel: w334 -> [_ w362]
          frame False {
          }
          frame True {
            n135 = property class="Pict"(reference=w366) -> (reference out=w361:refnum<vi>, "Value"=w365:picture)  [unwired: 1 in, 1 out]
            n136 = Array Size(array=w362) -> (size(s)=w358:i32)
            n137 = Search 1D Array(1D array=w362, element=w365) -> (index of element=w364:i32)  [unwired: 1 in]
            n138 = Increment(x=w364) -> (x+1=w359:i32)
            n139 = Quotient & Remainder(x=w359, y=w358) -> (x-y*floor(x/y)=w363:i32)  [unwired: 1 out]
            n140 = Index Array(array=w362, index=w363) -> (element=w360:picture)
            n141 = property class="Pict"(reference=w361, "Value"=w360) -> ()  [unwired: 1 in, 2 out]
          }
        }
        n142 = Replace Array Subset(array=w356, new element=1 ("new element/subarray"), index=w338) -> (w354:i32[])
        n143 = Subtract(x=w338, y=5) -> (x-y=w351:i32)
        n144 = Increment(x=w338) -> (x+1=w343:i32)
        n145 = Increment(x=w338) -> (x+1=w329:i32)
        n146 = Increment(x=w338) -> (x+1=w353:i32)
        n147 = property class="Slide (strict)"(reference=w344, "Value"=w343) -> ()  [unwired: 1 in, 2 out]
        n148 = Max & Min(x=w351, y=0) -> (max(x,y)=w349:i32)  [unwired: 1 out]
        n149 = Index Array(array=w345, index=w329) -> (element=w341:string)
        n150 = property on="Property Node" class="LstBox (strict)"(reference=w348, error in=w347, "Top Row"=w349, "Item Symbols"=w354, "Value"=w353) -> ()  [unwired: 2 out]
        n151 = property class="Str"(reference=w342, "Value"=w341) -> ()  [unwired: 1 in, 2 out]
        n152 = call <vilib>:"Add State(s) to Queue__JKI_lib_State_Machine.vi"("State(s) in (\"\")"=w330) -> ("States Out"=w331:string)  [unwired: 14 in]
      }
      frame "---------- Macro ----------" {
        # "Do not put any code in this frame.\n(It is a separator no-op. You can make a copy of this frame to create a new Macro frame)"
        n153 = call <vilib>:"Add State(s) to Queue__JKI_lib_State_Machine.vi"("State(s) in (\"\")"=w370) -> ("States Out"=w369:string)  [unwired: 14 in]
      }
      frame "Macro: Initialize" {
        # "Initialization Macro\n(This is called once, when the VI starts)"
        n154 = call <vilib>:"Add State(s) to Queue__JKI_lib_State_Machine.vi"("State(s) in Front (\"\")"="Data: Initialize\nData: InitializePolish\nInitialize Core Data\nData: List all lvclasses\nData: List all _JKI State Machine Helper VIs\nData: List all _JKI State Machine Helper Folders\nData: List all CSM Templates\nUI: Initialize\nUI: Front Panel State >> Open\nUI: Bring Window to Topmost(Windows Only)\nInitialize: Append steps of fixing JKISM Editor in MultiListbox\nInitialize: Append Simplify lvclass steps in Multilistbox\n//UI: Append Item to Multilistbox >> Refersh More Template palette\n//Initialize: Append Mass Compile Steps in MultiListbox\nInitialize: Append steps of et_csm_doc_case_as_default\n//github #330 https://github.com/NEVSTOP-LAB/Communicable-State-Machine/issues/330\n//Macro: Localize CSM\nMacro: Open VI for recompile\nInsert Task >> Refresh Popup Menus\nUI: Refresh Listbox\n\n//---------------\nMacro: Start\n//---------------\nMacro: Exit", "State(s) in (\"\")"=w375) -> ("States Out"=w374:string)  [unwired: 13 in]
      }
      frame "Macro: Start" {
        n155 = Unbundle By Name(w380) -> ("Actions"=w379:string[])
        n156 = call "CSM - Compact Multiple States.vi"("Multiple States"=w379) -> ("States"=w376:string)  [unwired: 9 in]
        n157 = call <vilib>:"Add State(s) to Queue__JKI_lib_State_Machine.vi"("State(s) in Front (\"\")"=w376, "State(s) in (\"\")"=w377) -> ("States Out"=w378:string)  [unwired: 13 in]
      }
      frame "Macro: Open VI for recompile" {
        n158 = Build Array("_xnode" ("name or relative path"), "_csmHelper" ("name or relative path"), "_popupMenuPlugin" ("name or relative path"), "_tool" ("name or relative path")) -> (w388:string[])
        n159 = for {
          tunnel: w388 -> [w404] mode=indexing
          tunnel: [w395] -> w389 mode=concatenating
          w396 = TRUE ("Treat LLBs as Folders?")
          n160 = call "CSM - user.lib Dir.vi"() -> ("csm_user.lib_dir"=w402:path)  [unwired: 2 in, 1 out]
          n161 = Build Path(base path=w402, name or relative path=w404) -> (appended path=w403:path)
          n162 = Path To String(path=w402) -> (string=w401:string)
          n163 = String Length(string=w401) -> (length=w400:i32)
          n164 = call <vilib>:"Recursive File List.vi"("pattern"="*.vi", "Continue Recursing on Error? (F)"=w396, "Treat LLBs as Folders?"=w396, "Folder Path"=w403) -> ("All Files in Dir"=w397:path[])  [unwired: 3 in, 4 out]
          n165 = for {
            tunnel: w397 -> [w412] mode=indexing
            tunnel: w400 -> [w410]
            tunnel: [w405] -> w398 mode=indexing
            n166 = Path To String(path=w412) -> (string=w411:string)
            n167 = String Subset(string=w411, offset (0)=w410) -> (substring=w409:string)  [unwired: 1 in]
            n168 = call <vilib>:"Build State String with Arguments__JKI_lib_State_Machine.vi"("Arguments (\"\")"=w409, "State"="Open VIRef to Compile CSM Tools") -> ("State with Arguments"=w407:string)  [unwired: 4 in]
            n169 = call <vilib>:"Build State String with Arguments__JKI_lib_State_Machine.vi"("Arguments (\"\")"=w407, "State"="Insert Task") -> ("State with Arguments"=w405:string)  [unwired: 4 in]
          }
          n170 = Reverse 1D Array(array=w398) -> (reversed array=w395:string[])
        }
        n171 = call "CSM - Compact Multiple States.vi"("Multiple States"=w389) -> ("States"=w385:string)  [unwired: 9 in]
        n172 = call <vilib>:"Add State(s) to Queue__JKI_lib_State_Machine.vi"("State(s) in (\"\")"="UI: Bring Window to Topmost(Windows Only)\nInsert Task >> Open VIRef to Compile CSM Tools2  >> user.lib\\_NEVSTOP\\Communicable State Machine(CSM)\\CSM User Interface(UI) Module Template.vi\nInsert Task >> Open VIRef to Compile CSM Tools2 >> user.lib\\_NEVSTOP\\Communicable State Machine(CSM)\\CSM Module Template.vi\nInsert Task >> Open VIRef to Compile CSM Tools2 >> templates\\Communicable State Machine(CSM)\\CSM DQMH-Style Template.vi\nInsert Task >> Open VIRef to Compile CSM Tools2 >> templates\\Communicable State Machine(CSM)\\CSM Module Template - Tiny.vi\nInsert Task >> Open VIRef to Compile CSM Tools2 >> templates\\Communicable State Machine(CSM)\\CSM User Interface(UI) Module Template - Tiny.vi" ("State(s) in Front (\"\")"), "State(s) at Back (\"\")"=w385) -> ("States Out"=w386:string)  [unwired: 13 in]
        n173 = call <vilib>:"Add State(s) to Queue__JKI_lib_State_Machine.vi"("State(s) in Front (\"\")"=w386, "State(s) in (\"\")"=w391) -> ("States Out"=w392:string)  [unwired: 13 in]
      }
      frame "Macro: Run CSM to Recompile" {
        n174 = call <vilib>:"Add State(s) to Queue__JKI_lib_State_Machine.vi"("State(s) in (\"\")"="Insert Task >> Run Template to Compile CSM API >> user.lib\\_NEVSTOP\\Communicable State Machine(CSM)\\CSM User Interface(UI) Module Template.vi\nInsert Task >> Run Template to Compile CSM API >> user.lib\\_NEVSTOP\\Communicable State Machine(CSM)\\CSM Module Template.vi\nInsert Task >> Run Template to Compile CSM API >> templates\\Communicable State Machine(CSM)\\CSM DQMH-Style Template.vi\nInsert Task >> Run Template to Compile CSM API >> templates\\Communicable State Machine(CSM)\\CSM Module Template - Tiny.vi\nInsert Task >> Run Template to Compile CSM API >> templates\\Communicable State Machine(CSM)\\CSM User Interface(UI) Module Template - Tiny.vi" ("State(s) in Front (\"\")")) -> ("States Out"=w413:string)  [unwired: 14 in]
        n175 = call <vilib>:"Add State(s) to Queue__JKI_lib_State_Machine.vi"("State(s) in Front (\"\")"=w413, "State(s) in (\"\")"=w415) -> ("States Out"=w416:string)  [unwired: 13 in]
      }
      frame "Macro: Localize CSM" {
        n176 = call <vilib>:"Add State(s) to Queue__JKI_lib_State_Machine.vi"("State(s) in (\"\")"="//Insert Task >> Check System Language\n//Insert Task >> Load Localization Files\n//Initialize: Localize All VIs\n//UI: Bring Window to Topmost(Windows Only)" ("State(s) in Front (\"\")")) -> ("States Out"=w419:string)  [unwired: 14 in]
        n177 = call <vilib>:"Add State(s) to Queue__JKI_lib_State_Machine.vi"("State(s) in Front (\"\")"=w419, "State(s) in (\"\")"=w421) -> ("States Out"=w422:string)  [unwired: 13 in]
      }
      frame "Macro: Exit" {
        # "Exit Macro\n(This is called once, when the VI exits)"
        n178 = Unbundle By Name(w431) -> ("Core.Close Panel on Exit?"=w430:bool)
        n179 = Select(t="UI: Front Panel State >> Close", s=w430, f="") -> (s? t:f=w427:string)
        n180 = call <vilib>:"Add State(s) to Queue__JKI_lib_State_Machine.vi"("State(s) in (\"\")"=w427, "State(s) at Back (\"\")"="Data: Cleanup\nExit") -> ("States Out"=w425:string)  [unwired: 13 in]
        n181 = call <vilib>:"Add State(s) to Queue__JKI_lib_State_Machine.vi"("State(s) in Front (\"\")"=w425, "State(s) in (\"\")"=w434) -> ("States Out"=w433:string)  [unwired: 13 in]
      }
      frame "---------------- Initialize ----------------" {
      }
      frame "Initialize: Append Recompile Steps in MultiListbox" {
        n182 = Unbundle By Name(w445) -> ("Actions"=w439:string[], "_JKI State Machine Helper VIs"=w444:path[])
        n183 = VI Library() -> (path=w442:path)
        n184 = Strip Path(path=w442) -> (stripped path=w441:path)  [unwired: 1 out]
        n185 = for {
          tunnel: w444 -> [w452] mode=indexing
          tunnel: [w448] -> w446 mode=indexing
          tunnel: w441 -> [w451]
          n186 = Path To String(path=w452) -> (string=w450:string)
          n187 = Path To String(path=w451) -> (string=w449:string)
          n188 = Search and Replace String(input string=w450, search string=w449) -> (result string=w453:string)  [unwired: 6 in, 3 out]
          n189 = Format Into String(format string="Recompile >> %s", w453) -> (resulting string=w448:string)  [unwired: 2 in, 1 out]
        }
        n190 = Build Array (concatenate)(w439, w446) -> (w438:string[])
        n191 = Bundle By Name(cluster=w445, "Actions"=w438) -> (w440:T3)
      }
      frame "Initialize: Append steps of fixing JKISM Editor in MultiListbox" {
        n192 = Unbundle By Name(w459) -> ("Actions"=w457:string[])
        n193 = Build Array (concatenate)(w457, string[] ["Fix JKISM Editor: fix_vi broken in Tree__JKI_State_Machine_Helper.vi", "Fix JKISM Editor: fix_Parse State Queue in Find Parse State Queue vi name.vi", "Fix JKISM Editor: fix_Parse State Queue in Find Parse State Queue vi name2.vi", "Fix JKISM Editor: Fix fix_exclude event case ref check.vi", "Fix JKISM Editor: fix_Find Event Stucture Ref vi.vi", "Fix JKISM Editor: fix_list event frames.vi"] ("element")) -> (w456:string[])
        n194 = Bundle By Name(cluster=w459, "Actions"=w456) -> (w458:T3)
      }
      frame "Initialize: Append Simplify lvclass steps in Multilistbox" {
        n195 = Unbundle By Name(w468) -> ("Actions"=w462:string[], "CSM lvclass"=w467:path[])
        n196 = call "CSM - user.lib Dir.vi"() -> ("<LabVIEW>"=w465:path)  [unwired: 2 in, 1 out]
        n197 = for {
          tunnel: w467 -> [w472] mode=indexing
          tunnel: [w477] -> w469 mode=indexing
          tunnel: w465 -> [w471]
          n198 = Path To String(path=w472) -> (string=w475:string)
          n199 = Path To String(path=w471) -> (string=w474:string)
          n200 = Search and Replace String(input string=w475, search string=w474) -> (result string=w473:string)  [unwired: 6 in, 3 out]
          n201 = Format Into String(format string="Clear lvclass mutation history >> %s", w473) -> (resulting string=w477:string)  [unwired: 2 in, 1 out]
        }
        n202 = Build Array (concatenate)(w462, w469) -> (w463:string[])
        n203 = Bundle By Name(cluster=w468, "Actions"=w463) -> (w464:T3)
      }
      frame "Initialize: Append Mass Compile Steps in MultiListbox" {
        n204 = Unbundle By Name(w486) -> ("Actions"=w480:string[], "_JKI State Machine Helper Folders"=w485:path[])
        n205 = VI Library() -> (path=w483:path)
        n206 = Strip Path(path=w483) -> (stripped path=w482:path)  [unwired: 1 out]
        n207 = for {
          tunnel: w485 -> [w492] mode=indexing
          tunnel: [w488] -> w478 mode=indexing
          tunnel: w482 -> [w491]
          n208 = Path To String(path=w492) -> (string=w490:string)
          n209 = Path To String(path=w491) -> (string=w489:string)
          n210 = Search and Replace String(input string=w490, search string=w489) -> (result string=w493:string)  [unwired: 6 in, 3 out]
          n211 = Format Into String(format string="Mass Compile >> %s", w493) -> (resulting string=w488:string)  [unwired: 2 in, 1 out]
        }
        n212 = Build Array (concatenate)(w480, w478) -> (w479:string[])
        n213 = Bundle By Name(cluster=w486, "Actions"=w479) -> (w481:T3)
      }
      frame "Initialize: Append steps of et_csm_doc_case_as_default" {
        n214 = Unbundle By Name(w501) -> ("Actions"=w495:string[], "CSM Templates"=w500:path[])
        n215 = call "CSM - user.lib Dir.vi"() -> ("<LabVIEW>"=w498:path)  [unwired: 2 in, 1 out]
        n216 = for {
          tunnel: w500 -> [w507] mode=indexing
          tunnel: [w504] -> w502 mode=indexing
          tunnel: w498 -> [w506]
          n217 = Path To String(path=w507) -> (string=w509:string)
          n218 = Path To String(path=w506) -> (string=w508:string)
          n219 = Search and Replace String(input string=w509, search string=w508) -> (result string=w505:string)  [unwired: 6 in, 3 out]
          n220 = Format Into String(format string="Set First CSM Case >> %s", w505) -> (resulting string=w504:string)  [unwired: 2 in, 1 out]
        }
        n221 = Build Array (concatenate)(w495, w502) -> (w496:string[])
        n222 = Bundle By Name(cluster=w501, "Actions"=w496) -> (w497:T3)
      }
      frame "Initialize: Append Item to Multilistbox", "Insert Task" {
        n223 = Unbundle By Name(w515) -> ("Actions"=w513:string[])
        n224 = Build Array(w517) -> (w516:string[])
        n225 = Build Array (concatenate)(w513, w516) -> (w512:string[])
        n226 = Bundle By Name(cluster=w515, "Actions"=w512) -> (w514:T3)
      }
      frame "Initialize: Localize All VIs" {
        n227 = call "CSM - user.lib Dir.vi"() -> ("<LabVIEW>"=w522:path)  [unwired: 2 in, 1 out]
        n228 = Unbundle By Name(w530) -> ("Actions"=w526:string[])
        n229 = Path to Array of Strings(0:w522) -> (2:w524:string[])  [unwired: 1 out]
        n230 = call "_list_CSM documented VIs.vi"() -> ("Array"=w525:path[])  [unwired: 11 in]
        n231 = Array Size(array=w524) -> (size(s)=w523:i32)
        n232 = for {
          tunnel: w525 -> [w538] mode=indexing
          tunnel: w523 -> [w536]
          tunnel: [w535] -> w521 mode=indexing
          n233 = Path to Array of Strings(0:w538) -> (2:w537:string[])  [unwired: 1 out]
          n234 = Array Subset(array=w537, index=w536) -> (w534:string[])  [unwired: 1 in]
          n235 = Array of Strings to Path(0:w534, 1:TRUE ("relative")) -> (2:w535:path)
        }
        n236 = Path To String(path=w521) -> (string=w519:string[])
        n237 = for {
          tunnel: [w541] -> w531 mode=indexing
          tunnel: "Localize VI Description >> %s" ("format string") -> [w540]
          tunnel: w519 -> [w539] mode=indexing
          n238 = Format Into String(format string=w540, w539) -> (resulting string=w541:string)  [unwired: 2 in, 1 out]
        }
        n239 = Build Array (concatenate)(w526, w531) -> (w527:string[])
        n240 = Bundle By Name(cluster=w530, "Actions"=w527) -> (w528:T3)
      }
      frame "---------- Action ----------" {
        # "Template Separator\n(You can make a copy of, or modify, this frame)"
        n241 = call <vilib>:"Add State(s) to Queue__JKI_lib_State_Machine.vi"("State(s) in (\"\")"=w545) -> ("States Out"=w544:string)  [unwired: 14 in]
      }
      frame "Recompile" {
        n242 = String To Path(string=w550) -> (path=w549:path)
        n243 = Open VI Reference(vi path=w549) -> (vi reference=w556:refnum<vi>, error out=w557:errorcluster)  [unwired: 5 in]
        n244 = invoke class="VI" method="Compile"(reference=w556, error in=w557, "Entire Hierarchy"=FALSE ("Compile Entire Hierarchy (F)"), "Force Compile"=TRUE ("Force Compile (T)")) -> (reference out=w555:refnum<vi>, error out=w554:errorcluster)  [unwired: 1 in, 3 out]
        n245 = invoke class="VI" method="Save.Instrument"(reference=w555, error in=w554) -> (reference out=w552:refnum<vi>, error out=w553:errorcluster)  [unwired: 4 in, 4 out]
        n246 = Close Reference(reference=w552, error in (no error)=w553) -> (error out=w551:errorcluster)
        n247 = call <vilib>:"Clear Errors.vi"("error in (no error)"=w551) -> ()  [unwired: 5 in, 2 out]
        n248 = call <vilib>:"Add State(s) to Queue__JKI_lib_State_Machine.vi"("State(s) in Front (\"\")"="UI: Post Action" ("State(s) in Front (\"\")"), "State(s) in (\"\")"=w547) -> ("States Out"=w548:string)  [unwired: 13 in]
      }
      frame "Set First CSM Case" {
        n249 = Match Pattern(string=w562, regular expression="^[\\\\]*") -> (before substring=w563:string)  [unwired: 1 in, 3 out]
        n250 = call "CSM - user.lib Dir.vi"() -> ("<LabVIEW>"=w566:path)  [unwired: 2 in, 1 out]
        n251 = Build Path(base path=w566, name or relative path=w563) -> (appended path=w565:path)
        n252 = call "_script_set_csm_doc_case_as_default.vi"("Vi Path"=w565) -> ("error out"=w570:errorcluster)  [unwired: 10 in]
        n253 = call <vilib>:"Clear Errors.vi"("error in (no error)"=w570) -> ()  [unwired: 5 in, 2 out]
        n254 = call <vilib>:"Add State(s) to Queue__JKI_lib_State_Machine.vi"("State(s) in Front (\"\")"="UI: Post Action" ("State(s) in Front (\"\")"), "State(s) in (\"\")"=w568) -> ("States Out"=w569:string)  [unwired: 13 in]
      }
      frame "Clear lvclass mutation history" {
        n255 = Match Pattern(string=w573, regular expression="^[\\\\]*") -> (before substring=w574:string)  [unwired: 1 in, 3 out]
        n256 = call "CSM - user.lib Dir.vi"() -> ("<LabVIEW>"=w577:path)  [unwired: 2 in, 1 out]
        n257 = Build Path(base path=w577, name or relative path=w574) -> (appended path=w576:path)
        n258 = call "clear the mutation history for the classes.vi"("Path"=w576) -> ()  [unwired: 11 in]
        n259 = call <vilib>:"Add State(s) to Queue__JKI_lib_State_Machine.vi"("State(s) in Front (\"\")"="UI: Post Action" ("State(s) in Front (\"\")"), "State(s) in (\"\")"=w579) -> ("States Out"=w580:string)  [unwired: 13 in]
      }
      frame "Fix JKISM Editor: fix_Parse State Queue in Find Parse State Queue vi name.vi" {
        n260 = call "_script_fix_Parse State Queue in Find Parse State Queue vi name.vi"() -> ()  [unwired: 12 in]
        n261 = call <vilib>:"Add State(s) to Queue__JKI_lib_State_Machine.vi"("State(s) in Front (\"\")"="UI: Post Action" ("State(s) in Front (\"\")"), "State(s) in (\"\")"=w584) -> ("States Out"=w585:string)  [unwired: 13 in]
      }
      frame "Fix JKISM Editor: fix_Parse State Queue in Find Parse State Queue vi name2.vi" {
        n262 = call "_script_fix_Parse State Queue in Find Parse State Queue vi name2.vi"() -> ()  [unwired: 12 in]
        n263 = call <vilib>:"Add State(s) to Queue__JKI_lib_State_Machine.vi"("State(s) in Front (\"\")"="UI: Post Action" ("State(s) in Front (\"\")"), "State(s) in (\"\")"=w589) -> ("States Out"=w590:string)  [unwired: 13 in]
      }
      frame "Fix JKISM Editor: fix_vi broken in Tree__JKI_State_Machine_Helper.vi" {
        n264 = call "_script_fix_vi broken in Tree__JKI_State_Machine_Helper.vi"() -> ()  [unwired: 12 in]
        n265 = call <vilib>:"Add State(s) to Queue__JKI_lib_State_Machine.vi"("State(s) in Front (\"\")"="UI: Post Action" ("State(s) in Front (\"\")"), "State(s) in (\"\")"=w594) -> ("States Out"=w595:string)  [unwired: 13 in]
      }
      frame "Fix JKISM Editor: Fix fix_exclude event case ref check.vi" {
        n266 = call "_script_fix_exclude event case ref check.vi"() -> ()  [unwired: 12 in]
        n267 = call <vilib>:"Add State(s) to Queue__JKI_lib_State_Machine.vi"("State(s) in Front (\"\")"="UI: Post Action" ("State(s) in Front (\"\")"), "State(s) in (\"\")"=w599) -> ("States Out"=w600:string)  [unwired: 13 in]
      }
      frame "Fix JKISM Editor: fix_Find Event Stucture Ref vi.vi" {
        n268 = call "_script_fix_Find Event Stucture Ref vi.vi"() -> ()  [unwired: 12 in]
        n269 = call <vilib>:"Add State(s) to Queue__JKI_lib_State_Machine.vi"("State(s) in Front (\"\")"="UI: Post Action" ("State(s) in Front (\"\")"), "State(s) in (\"\")"=w604) -> ("States Out"=w605:string)  [unwired: 13 in]
      }
      frame "Fix JKISM Editor: fix_list event frames.vi" {
        n270 = call "_script_fix_list event frames.vi"() -> ()  [unwired: 12 in]
        n271 = call <vilib>:"Add State(s) to Queue__JKI_lib_State_Machine.vi"("State(s) in Front (\"\")"="UI: Post Action" ("State(s) in Front (\"\")"), "State(s) in (\"\")"=w609) -> ("States Out"=w610:string)  [unwired: 13 in]
      }
      frame "Mass Compile" {
        n272 = Match Pattern(string=w613, regular expression="^[\\\\]*") -> (before substring=w614:string)  [unwired: 1 in, 3 out]
        n273 = call "CSM - user.lib Dir.vi"() -> ("<LabVIEW>"=w617:path)  [unwired: 2 in, 1 out]
        n274 = Build Path(base path=w617, name or relative path=w614) -> (appended path=w616:path)
        n275 = invoke class="App" method="Mass Compile"("Directory to Compile"=w616) -> (error out=w623:errorcluster)  [unwired: 8 in, 8 out]
        n276 = call <vilib>:"Clear Errors.vi"("error in (no error)"=w623) -> ()  [unwired: 5 in, 2 out]
        n277 = Wait (ms)(milliseconds to wait=u32 1000) -> ()  [unwired: 1 out]
        n278 = call <vilib>:"Add State(s) to Queue__JKI_lib_State_Machine.vi"("State(s) in Front (\"\")"="UI: Post Action" ("State(s) in Front (\"\")"), "State(s) in (\"\")"=w619) -> ("States Out"=w620:string)  [unwired: 13 in]
      }
      frame "Run Template to Compile CSM API" {
        n279 = call "CSM - user.lib Dir.vi"() -> ("<LabVIEW>"=w625:path)  [unwired: 2 in, 1 out]
        n280 = Build Path(base path=w625, name or relative path=w626) -> (appended path=w629:path)
        n281 = call <vilib>:"Check if File or Folder Exists.vi"("path"=w629) -> ("file or folder exists?"=w627:bool, "dup path"=w628:path)  [unwired: 8 in, 1 out]
        n282 = case shown="True" w627 {
          tunnel: w628 -> [w635 w638]
          frame False {
            n283 = Path To String(path=w635) -> (string=w636:string)
            n284 = Two Button Dialog(message=w636, 2:"Ack" ("T button name (\"OK\")")) -> ()  [unwired: 1 in, 1 out]
          }
          frame True {
            n285 = call "uuid.vi"() -> ("UUID"=w641:string)  [unwired: 11 in]
            n286 = Open VI Reference(type specifier VI Refnum (for type only)=refnum<vi> refnum, vi path=w638, options=128) -> (vi reference=w645:refnum<vi>, error out=w646:errorcluster)  [unwired: 3 in]
            n287 = call-by-ref "Start Asynchronous Call"(reference=w645, error in=w646, "Name(\"\" to use uuid)"=w641) -> (reference out=w648:refnum<vi>, error out=w647:errorcluster)  [unwired: 11 in]
            n288 = Close Reference(reference=w648, error in (no error)=w647) -> (error out=w643:errorcluster)
            n289 = flat-sequence {
              tunnel: w643 -> [w650]
              tunnel: [w650] -> w642
              frame #0 {
                n290 = Wait (ms)(milliseconds to wait=u32 500) -> ()  [unwired: 1 out]
              }
            }
            n291 = call "CSM - Send Message and Wait for Reply.vi"("Error In (No Error)"=w642, "Target Module"=w641, "State"="Macro: Exit") -> ("error out"=w639:errorcluster)  [unwired: 6 in, 2 out]
            n292 = call <vilib>:"Clear Errors.vi"("error in (no error)"=w639) -> ()  [unwired: 5 in, 2 out]
          }
        }
        n293 = call <vilib>:"Add State(s) to Queue__JKI_lib_State_Machine.vi"("State(s) in Front (\"\")"="UI: Post Action" ("State(s) in Front (\"\")"), "State(s) in (\"\")"=w631) -> ("States Out"=w632:string)  [unwired: 13 in]
      }
      frame "Open VIRef to Compile CSM Tools" {
        n294 = Match Pattern(string=w654, regular expression="^[\\\\]*") -> (after substring=w652:string)  [unwired: 1 in, 3 out]
        n295 = call "CSM - user.lib Dir.vi"() -> ("csm_user.lib_dir"=w658:path)  [unwired: 2 in, 1 out]
        n296 = Build Path(base path=w658, name or relative path=w652) -> (appended path=w659:path)
        n297 = call <vilib>:"Check if File or Folder Exists.vi"("path"=w659) -> ("error out"=w657:errorcluster, "file or folder exists?"=w656:bool, "dup path"=w655:path)  [unwired: 8 in]
        n298 = case shown="False" w656 {
          tunnel: w657 -> [_ w670]
          tunnel: w655 -> [w666 w669]
          frame False {
            n299 = Path To String(path=w666) -> (string=w665:string)
            n300 = Two Button Dialog(message=w665, 2:"Ack" ("T button name (\"OK\")")) -> ()  [unwired: 1 in, 1 out]
          }
          frame True {
            n301 = Open VI Reference(vi path=w669, options=2, error in (no error)=w670) -> (vi reference=w671:refnum<vi>, error out=w675:errorcluster)  [unwired: 3 in]
            n302 = flat-sequence {
              tunnel: w675 -> [w679]
              tunnel: [w678] -> w674
              tunnel: [w676] -> w672
              tunnel: w671 -> [w677]
              frame #0 {
                n303 = invoke class="VI" method="Save.Instrument"(reference=w677, error in=w679) -> (reference out=w676:refnum<vi>, error out=w678:errorcluster)  [unwired: 4 in, 4 out]
                n304 = Wait (ms)(milliseconds to wait=u32 50) -> ()  [unwired: 1 out]
              }
            }
            n305 = Close Reference(reference=w672, error in (no error)=w674) -> (error out=w673:errorcluster)
            n306 = call <vilib>:"Clear Errors.vi"("error in (no error)"=w673) -> ()  [unwired: 5 in, 2 out]
          }
        }
        n307 = call <vilib>:"Add State(s) to Queue__JKI_lib_State_Machine.vi"("State(s) in Front (\"\")"="UI: Post Action" ("State(s) in Front (\"\")"), "State(s) in (\"\")"=w661) -> ("States Out"=w662:string)  [unwired: 13 in]
      }
      frame "Open VIRef to Compile CSM Tools2" {
        n308 = Match Pattern(string=w684, regular expression="^[\\\\]*") -> (after substring=w682:string)  [unwired: 1 in, 3 out]
        n309 = call "CSM - user.lib Dir.vi"() -> ("<LabVIEW>"=w681:path)  [unwired: 2 in, 1 out]
        n310 = Build Path(base path=w681, name or relative path=w682) -> (appended path=w688:path)
        n311 = call <vilib>:"Check if File or Folder Exists.vi"("path"=w688) -> ("error out"=w687:errorcluster, "file or folder exists?"=w686:bool, "dup path"=w685:path)  [unwired: 8 in]
        n312 = case shown="True" w686 {
          tunnel: w687 -> [_ w699]
          tunnel: w685 -> [w695 w698]
          frame False {
            n313 = Path To String(path=w695) -> (string=w694:string)
            n314 = Two Button Dialog(message=w694, 2:"Ack" ("T button name (\"OK\")")) -> ()  [unwired: 1 in, 1 out]
          }
          frame True {
            n315 = Open VI Reference(vi path=w698, options=2, error in (no error)=w699) -> (vi reference=w700:refnum<vi>, error out=w704:errorcluster)  [unwired: 3 in]
            n316 = flat-sequence {
              tunnel: w704 -> [w708]
              tunnel: [w707] -> w703
              tunnel: [w705] -> w701
              tunnel: w700 -> [w706]
              frame #0 {
                n317 = invoke class="VI" method="Save.Instrument"(reference=w706, error in=w708) -> (reference out=w705:refnum<vi>, error out=w707:errorcluster)  [unwired: 4 in, 4 out]
                n318 = Wait (ms)(milliseconds to wait=u32 50) -> ()  [unwired: 1 out]
              }
            }
            n319 = Close Reference(reference=w701, error in (no error)=w703) -> (error out=w702:errorcluster)
            n320 = call <vilib>:"Clear Errors.vi"("error in (no error)"=w702) -> ()  [unwired: 5 in, 2 out]
          }
        }
        n321 = call <vilib>:"Add State(s) to Queue__JKI_lib_State_Machine.vi"("State(s) in Front (\"\")"="UI: Post Action" ("State(s) in Front (\"\")"), "State(s) in (\"\")"=w690) -> ("States Out"=w691:string)  [unwired: 13 in]
      }
      frame "Refresh Popup Menus" {
        n322 = VI Library() -> (path=w718:path)
        n323 = Strip Path(path=w718) -> (stripped path=w717:path)  [unwired: 1 out]
        n324 = Build Path(base path=w717, name or relative path="resource\\plugins\\PopupMenus\\support\\Refresh Menus.vi") -> (appended path=w715:path)
        n325 = call <vilib>:"Check if File or Folder Exists.vi"("path"=w715) -> ("file or folder exists?"=w713:bool, "dup path"=w714:path)  [unwired: 8 in, 1 out]
        n326 = case shown="True" w713 {
          tunnel: w714 -> [_ w727]
          frame False {
          }
          frame True {
            n327 = Open VI Reference(vi path=w727) -> (vi reference=w726:refnum<vi>, error out=w725:errorcluster)  [unwired: 5 in]
            n328 = invoke class="VI" method="Run VI"(reference=w726, error in=w725, "Wait until done"=TRUE ("Wait Until Done"), "Auto Dispose Ref"=FALSE ("Auto Dispose Reference")) -> (reference out=w721:refnum<vi>, error out=w722:errorcluster)  [unwired: 1 in, 3 out]
            n329 = Close Reference(reference=w721, error in (no error)=w722) -> ()  [unwired: 1 out]
          }
        }
        n330 = call <vilib>:"Add State(s) to Queue__JKI_lib_State_Machine.vi"("State(s) in Front (\"\")"="UI: Post Action" ("State(s) in Front (\"\")"), "State(s) in (\"\")"=w711) -> ("States Out"=w712:string)  [unwired: 13 in]
      }
      frame "Check System Language" {
        n331 = call "_csm_System_Language.vi"() -> ("LangID"=w731:string)  [unwired: 11 in]
        n332 = Bundle By Name(cluster=w733, "LangID"=w731) -> (w732:T3)
        n333 = call <vilib>:"Add State(s) to Queue__JKI_lib_State_Machine.vi"("State(s) in Front (\"\")"="UI: Post Action" ("State(s) in Front (\"\")"), "State(s) in (\"\")"=w729) -> ("States Out"=w730:string)  [unwired: 13 in]
      }
      frame "Load Localization Files" {
        w735 = variant ("DescMap")
        n334 = Unbundle By Name(w740) -> ()  [unwired: 1 out]
        n335 = call "CSM - user.lib Dir.vi"() -> ("<LabVIEW>"=w741:path)  [unwired: 2 in, 1 out]
        n336 = Build Path(base path=w741, name or relative path="help\\NEVSTOP\\Communicable State Machine(CSM)") -> ()  [unwired: 1 out]
        n337 = Bundle By Name(cluster=w740, "DescMap"=w735, "NoteMap"=w735) -> (w739:T3)
        n338 = call <vilib>:"Add State(s) to Queue__JKI_lib_State_Machine.vi"("State(s) in Front (\"\")"="UI: Post Action" ("State(s) in Front (\"\")"), "State(s) in (\"\")"=w737) -> ("States Out"=w738:string)  [unwired: 13 in]
      }
      frame "Localize VI Description" {
        n339 = Unbundle By Name(w751) -> ("LangID"=w752:string, "DescMap"=w754:variant, "NoteMap"=w755:variant)
        n340 = call "CSM - user.lib Dir.vi"() -> ("<LabVIEW>"=w756:path)  [unwired: 2 in, 1 out]
        n341 = Match Pattern(string=w745, regular expression="^[\\\\]*") -> (before substring=w744:string)  [unwired: 1 in, 3 out]
        n342 = Build Path(base path=w756, name or relative path=w744) -> (appended path=w753:path)
        n343 = Strip Path(path=w753) -> (name=w761:string)  [unwired: 1 out]
        n344 = Get Variant Attribute(Variant=w754, name=w761, default value (empty Variant)="" ("String")) -> (found=w760:bool, value=w757:string, error out=w759:errorcluster)  [unwired: 1 in, 1 out]
        n345 = case shown="True" w760 {
          tunnel: w759 -> [w762 w765]
          tunnel: [w762 w766] -> w750
          tunnel: w757 -> [_ w763]
          tunnel: w755 -> [_ _]
          tunnel: w753 -> [_ w764]
          tunnel: w752 -> [_ _]
          frame False {
          }
          frame True {
            n346 = call "Populate Single VI Help.vi"("error in (no error)"=w765, "VI Description"=w763, "Path"=w764) -> ("error out"=w766:errorcluster)  [unwired: 8 in]
          }
        }
        n347 = call <vilib>:"Add State(s) to Queue__JKI_lib_State_Machine.vi"("State(s) in Front (\"\")"="UI: Post Action" ("State(s) in Front (\"\")"), "State(s) in (\"\")"=w748) -> ("States Out"=w749:string)  [unwired: 13 in]
      }
    }
  }
  n348 = call <vilib>:"Clear Errors.vi"("error in (no error)"=w1) -> ()  [unwired: 5 in, 2 out]
